vi "1_WF_Anomaly_Detection(Training).vi"() -> ()   [LabVIEW 2020]
doc: "Demonstrates the usage of Deep Learning Toolkit for solving hand written digit recognition problem with multilayer perceptron (MLP).\nDataset: MNIST http://yann.lecun.com/exdb/mnist/\nRequirements: Deep Learning Toolkit for LabVIEW"
uses:
  <vilib>/Ngene/Deep Learning Toolkit/Toolkit/NN_Train/Controls/NN_Train_Session_Data.ctl
  <vilib>/Ngene/Deep Learning Toolkit/Toolkit/NN_Train/Controls/NN_LR_Policy_Cfg.ctl
  <vilib>/Ngene/Deep Learning Toolkit/Toolkit/NN_Train/Controls/NN_LR_Policy_Type.ctl
  <vilib>/Ngene/Deep Learning Toolkit/Toolkit/NN_Train/Controls/NN_Train_Params.ctl
  <vilib>/Ngene/Deep Learning Toolkit/Toolkit/NN_Train/Controls/NN_Train_Optimizer.ctl
  <vilib>/Ngene/Deep Learning Toolkit/Toolkit/NN_Train/Controls/NN_Train_Data_Sampling.ctl
  <vilib>/Ngene/Deep Learning Toolkit/Toolkit/NN_Network/Controls/NN_Device.ctl
  <vilib>/Ngene/Deep Learning Toolkit/Toolkit/NN_Layers/Layers/Input/Controls/NN_Layer_Config_Aug(Input1D).ctl
  <vilib>/Ngene/Deep Learning Toolkit/Toolkit/NN_Layers/Layers/Input/Controls/Aug/NN_Input1D_Aug_Config.ctl
  <vilib>/Ngene/Deep Learning Toolkit/Toolkit/NN_Layers/Layers/Input/Controls/Aug/NN_Input1D_Aug_Types.ctl
  <vilib>/Ngene/Deep Learning Toolkit/Toolkit/NN_Layers/Layers/Input/Controls/Aug/Aug_Distribution_Type.ctl
  <vilib>/Ngene/Deep Learning Toolkit/Toolkit/NN_Layers/Layers/FC/Controls/NN_Layer_Config(FC).ctl
  <vilib>/Ngene/Deep Learning Toolkit/Toolkit/NN_Layers/Layers/BatchNorm/Controls/NN_BN_Params.ctl
  <vilib>/Ngene/Deep Learning Toolkit/Toolkit/NN_Activations/Controls/NN_Activation_Type.ctl
  <vilib>/Ngene/Deep Learning Toolkit/Toolkit/NN_Layers/Controls/NN_Layer_Init_Params.ctl
  <vilib>/Ngene/Deep Learning Toolkit/Toolkit/NN_Layers/Controls/NN_Layer_Weight_Init_Type.ctl
  <vilib>/Ngene/Deep Learning Toolkit/Toolkit/NN_Layers/Layers/Input/Controls/NN_Layer_Config(Input1D).ctl
  <vilib>/Ngene/Deep Learning Toolkit/Toolkit/NN_Data/Controls/NN_Data_type.ctl
  <vilib>/Ngene/Deep Learning Toolkit/Toolkit/NN_Network/Controls/NN_Save_Before_Destroy_Options.ctl
  <vilib>/Ngene/Deep Learning Toolkit/Toolkit/NN_Layers/Layers/FC/NN_Layer_Create(FC).vi
  <vilib>/Ngene/Deep Learning Toolkit/Toolkit/NN_Layers/Layers/Input/NN_Layer_Create(Input1D).vi
  <vilib>/Ngene/Deep Learning Toolkit/Toolkit/NN_Data/subVIs/Dataset/NN_Variant_to_DVR/2D/NN_Data_Variant_to_DVR(2D_SGL).vi
  <vilib>/Ngene/Deep Learning Toolkit/Toolkit/NN_Train/SubVIs/Dataset_Checks/NN_Check_Dataset(In1D_Out1D).vi
  <vilib>/Ngene/Deep Learning Toolkit/Toolkit/NN_Network/API/NN_Set_Input/1D/NN_Set_Input(1D_SGL_idx).vi
  <vilib>/Ngene/Deep Learning Toolkit/Toolkit/NN_Data/subVIs/Get_Data_Vals/2D/NN_Data_Get_ValByRef(2D_SGL_idx).vi
  <vilib>/Ngene/Deep Learning Toolkit/Toolkit/NN_Train/Loss_Functions/NN_Set_Loss(MSE).vi
  <vilib>/Ngene/Deep Learning Toolkit/Toolkit/Deep_Learning_Toolkit_by_Ngene.lvlib
  <vilib>/ptbypt/NI_PtbyPt.lvlib
panel:
  in  "Normal/Abnormal":bool=TRUE
  in  "Validation(Abnormal) dataset path":path=path "D:/working/Anomaly Detection/Validation/Abnormal"
  in  "Validation(Normal) dataset path":path=path "D:/working/Anomaly Detection/Validation/Normal"
  in  "Train(Normal) dataset path":path=path "D:/working/Anomaly Detection/Train/Normal"
  out "Anomaly Score":sgl[](graph)=[0.060092747, 0.057043016, 0.032625258, 0.00050622225, 0.07121873, 0.09103888, 0.0006431341, 0.04204446, 0.0002219677, 0.02923894, 0.060141027, 0.06411958, 0.064849555, 0.010767877, 0.033320367, 0.07314634, 0.035111904, 0.042108685, 0.01123029, 0.028102368, 0.024529666, 0.004258156, 0.024849623, 0.03586331, 0.024636567, 0.056010053, 0.006806895, 0.047554873, 0.07157735, 0.027011871, 0.025139395, 0.022341115, 0.032895457, 0.0022708364, 0.024684738, 0.006394863, 0.014353149, 0.018841192, 0.0883885, 0.048397973, 0.035732955, 0.06335908, 0.030065864, 0.03291616, 0.05862975, 0.041152924, 0.04338476, 0.00016877055, 0.009982914, 0.046630204, 0.04450816, 0.053127766, 0.03401476, 0.0791775, 0.04717928, 0.07712877, 0.058600783, 0.04143399, 0.08513886, 0.06798601, 0.051917136, 0.044983864, 0.10643387, 0.09333289, 0.10147804, 0.08439672, 0.065609634, 0.036409795, 0.073546946, 0.10952538, 0.055474997, 0.1068089, 0.084765375, 0.057112873, 0.054448366, 0.07403237, 0.06890768, 0.070016384, 0.053028703, 0.08037907, 0.04426396, 0.043441594, 0.08644903, 0.088015676, 0.047763288, 0.099104345, 0.048645973, 0.07637364, 0.014656782, 0.07575214, 0.05684656, 0.022864163, 0.017387092, 0.015441477, 0.06586057, 0.02807647, 0.018982649, 0.021074474, 0.026940286, 0.066253364, 0.018976212, 0.010368884, 0.020807803, 0.074733555, 0.019434988, 0.017290056, 0.015355766, 0.017493486, 0.033833265, 0.0105896, 0.044781208, 0.031580508, 0.009655416, 0.04107994, 0.03886822, 0.022953898, 0.015816778, 0.040687352, 0.01231581, 0.045750678, 0.0053392947, 0.021824911, 0.024692237, 0.006048307, 0.035785183, 0.0044120774, 0.024970394, 0.032739528, 0.02630835, 0.019736473, 0.10281274, 0.003404349, 0.10191603, 0.038091034, 0.03535904, 0.0002465546, 0.042997003, 0.04390773, 0.06490451, 0.09284058, 0.083866745, 0.084221035, 0.104360044, 0.04381025, 0.04932916, 0.06883395, 0.063578606, 0.05527377, 0.02474022, 0.0023239255, 0.09212524, 0.089194, 0.032360792, 0.06271982, 0.047680855, 0.050662935, 0.027425885, 0.06428027, 0.01801461, 0.04022503, 0.012174964, 0.068769336, 0.039433062, 0.03701794, 0.05450797, 0.069071054, 0.03687513, 0.0761683, 0.04485655, 0.046353817, 0.005211234, 0.03217846, 0.05994767, 0.021627009, 0.02824694, 0.025053084, 0.011249602, 0.013183653, 0.0628652, 0.033547223, 0.010532796, 0.071924865, 0.048714876, 0.025912106, 0.067157984, 0.057994485, 0.012352109, 0.03120172, 0.031498015, 0.0038321614, 0.005246043, 0.024365425, 0.07627022, 0.056759536, 0.0038585067, 0.0013263822, 0.035828173, 0.010404587, 0.06529927, 0.025035083, 0.012059271, 0.019346893, 0.026661277, 0.040283203, 0.043239236, 0.041656077, 0.011768699, 0.023633242, 0.035004884, 0.0050939023, 0.0053791404, 0.04120791, 0.0638271, 0.026579648, 0.00066304207, 0.0075542033, 0.013537571, 0.0042291284, 0.040332705, 0.020002171, 0.036556043, 0.009527139, 0.013155438, 0.01560469, 0.023518208, 0.0110270865, 0.010643028, 0.026360236, 0.02436541, 0.030391306, 0.050228402, 0.04228738, 0.0033869147, 0.036175907, 0.00611943, 0.08756912, 0.049255222, 0.020914257, 0.0037515163, 0.05814132, 0.022490084, 0.021241128, 0.036547303, 0.012504697, 0.056980252, 0.0651865, 0.04526204, 0.04104632, 0.020310044, 0.034356654, 0.0019336343, 0.064979196, 0.024666071, 0.07885355, 0.060456753, 0.057785153, 0.06992471, 0.024199843, 0.048030198, 0.061351597, 0.019730091, 0.03939289, 0.097007036, 0.0006953478, 0.008476853, 0.052414775, 0.0017266273, 0.036400378, 0.03022182, 0.06443, 0.0019540787, 0.0030147433, 0.0060815215, 0.03073597, 0.054870903, 0.0070074797, 0.029543698, 0.0017739534, 0.024344265, 0.058060706, 0.0073035955, 0.014600635, 0.0053038597, 0.024832547, 0.053949594, 0.031209469, 0.030771732, 0.036867917, 0.034106612, 0.018789113, 0.012063682, 0.024652004, 0.025159836, 0.018065631, 0.0015200973, 0.010810316, 0.02901429, 0.021046221, 0.04046935, 0.047151983, 0.073693275, 0.0008752346, 0.011598229, 0.02580303, 0.02341029, 0.014973015, 0.018914193, 0.00989604, 0.05237758, 0.043263435, 0.02045992, 0.014319763, 0.029384151, 0.03725402, 0.008532152, 0.021618426, 0.08714062, 0.012386654, 0.034504678, 0.05780665, 0.025059067, 0.037491217, 0.0035665482, 0.07386769, 0.006312445, 0.066935435, 0.08569892, 0.07021108, 0.04160881, 0.0135602355, 0.04307291, 0.017525911, 0.0078089833, 0.040077955, 0.06780583, 0.011282504, 0.027252495, 0.0052479506, 0.08056086, 0.051447213, 0.07204753, 0.045395255, 0.009712577, 0.00199759, 0.0043674707, 0.02886641, 0.057467997, 0.0033851862, 0.018882632, 0.035472095, 0.07547408, 0.05349207, 0.013515651, 0.023959875, 0.059220076, 0.028184414, 0.0042169094, 0.0054979324, 0.021413028, 0.00018376112, 0.04798007, 0.0035876632, 0.00085502863, 0.015411198, 0.03357798, 0.0141349435, 0.025293052, 0.06722516, 0.035633385, 0.03246671, 0.0073210597, 0.0033890605, 0.051241398, 0.031478405, 0.0120385885, 0.04314059, 0.0051404834, 0.0022211075, 0.060732722, 0.03339243, 0.027571142, 0.03379011, 0.02301824, 0.023383796, 0.023100555, 0.0034759045, 0.004920721, 0.014518559, 0.005325496, 0.06771225, 0.029369414, 0.037244976, 0.028220832, 0.035060287, 0.019271076, 0.045505702, 0.06212762, 0.037652284, 0.012569755, 0.012304664, 0.046938777, 0.029604435, 0.016992986, 0.02305895, 0.0012228787, 0.014539182, 0.016175747, 0.041780204, 0.032874674, 0.04862517, 0.07770675, 0.04169628, 0.058294393, 0.053397845, 0.07256114, 0.033954605, 0.060890388, 0.0009793043, 0.109390326, 0.048723236, 0.006696999, 0.013124093, 0.03138551, 0.02865538, 0.0050074756, 0.026816845, 0.0021244586, 0.01151374, 0.010649353, 0.036117435, 0.01668498, 0.041314363, 0.03689885, 0.011788726, 0.04051286, 0.048635185, 0.0010183454, 0.03554952, 0.049126625, 0.049170673, 0.04226947, 0.02651894, 0.026122332, 0.00902319, 0.014714181, 0.053105295, 0.03526801, 0.045228064, 0.005509317, 0.012253821, 0.008698344, 0.02798599, 0.03927982, 0.009805262, 0.023320377, 0.026049614, 0.030642271, 0.0005450845, 0.0044911504, 0.013210893, 0.025141537, 0.027490556, 0.011119723, 0.027630031, 0.013084769, 0.037715316, 0.01857531, 0.0246706, 0.028110027, 0.017253816, 0.055761278, 0.02272594, 0.02098006, 0.023195267, 0.008237243, 0.034432173, 0.03778249, 0.0037900805, 0.016308367, 0.01734817, 0.05744642, 0.044672668, 0.014907718, 0.02106911, 0.022406042, 0.0028811693, 0.048549235, 0.07803196, 0.043880284, 0.007881284, 0.014288545, 0.040141463, 0.037219048, 0.025383472, 0.028543562, 0.037507176, 0.06284988, 0.06856242, 0.045178384, 0.06358957, 0.06256491, 0.09023467, 0.066772714, 0.03930801, 0.089330375, 0.045202382, 0.0012217015, 0.03294455, 0.074084684, 0.031060789, 0.07108601, 0.06460565, 0.03949655, 0.02086892, 0.022628829, 0.0531967, 0.043416634, 3.7267804e-05, 0.0069933236, 0.007908642, 0.00840199, 0.010333836, 0.08059165, 0.018291354, 0.00983268, 0.02023545, 0.052577674, 0.028196096, 0.04909426, 0.06960064, 0.018643081, 0.018747628, 0.052239835, 0.03520423, 0.020172, 0.035363674, 0.03190261, 0.03205198, 0.027214646, 0.0010645986, 0.033943415, 0.06383264, 0.026733339, 0.023622096, 0.006123543, 0.034471333, 0.0123743415, 0.037702322, 0.022325516, 0.0033456087, 0.015103638, 0.038256645, 0.00042706728, 0.032328308, 0.0027711987, 0.029803038, 0.029901206, 0.016103625, 0.040743887, 0.020637393, 0.032048166, 0.017939508, 0.03243172, 0.0057141185, 0.012813866, 0.013404548, 0.012252271, 0.0017794967, 0.0056546926, 0.04450822, 0.05620414, 0.013124406, 0.018638313, 0.022311866, 0.030828714, 0.06490421, 0.046281636, 0.057371557, 0.03398019, 0.01053822, 0.022645772, 0.050679624, 0.02049148, 0.02902317, 0.059186637, 0.031636357, 0.0341025, 0.003514707, 0.034976006, 0.050084323, 0.06393728, 0.027762264, 0.030045897, 0.0034492016, 0.04939601, 0.026292771, 0.03334993, 0.016023219, 0.055217057, 0.08875525, 0.034162715, 0.03684184, 0.09832852, 0.0032533929, 0.04504199, 0.072000064, 0.008023124, 0.03721671, 0.07505199, 0.07275631, 0.061018378, 0.033247128, 0.04330583, 0.016284913, 0.07300937, 0.05863276, 0.060104758, 0.015596688, 0.020811826, 0.056227475, 0.109434426, 0.050217718, 0.011233985, 0.016816437, 0.014317572, 0.017227054, 0.01705122, 0.067214906, 0.007261336, 0.0041286945, 0.004626453, 0.008798957, 0.033632636, 0.011648834, 0.0064768195, 0.015599787, 0.010294795, 0.03991133, 0.022496164, 0.01535368, 0.010416925, 0.014266193, 0.004371822, 0.05693829, 0.03694272, 0.01812011, 0.008884549, 0.014544427, 0.01466769, 0.014502704, 0.03141892, 0.004409075, 0.01927048, 0.0057350993, 0.010116279, 0.010567248, 0.02657038, 0.03631872, 0.02690959, 0.004686594, 0.033815324, 0.016802311, 0.0529083, 0.018151581, 0.04130584, 0.008548856, 0.049080312, 0.0076634884, 0.021098077, 0.011823714, 0.0067802668, 0.018489897, 0.022878766, 0.041176736, 0.042533934, 0.06584221, 0.02490908, 0.054923594, 0.052935958, 0.01268357, 0.06410545, 0.05014521, 0.046426475, 0.020729423, 0.026006311, 0.04061067, 0.032135606, 0.01457727, 0.04491949, 0.08099672, 0.020792186, 0.018885136, 0.013119906, 0.00464952, 0.036944523, 0.022346139, 0.0232165, 0.048607357, 0.06732133, 0.026639529, 0.042294167, 0.059899196, 0.04408887, 0.056200996, 0.022303723, 0.026353091, 0.025170714, 0.011349812, 0.027633563, 0.07789123, 0.039173394, 0.026246369, 0.0060180426, 0.058868974, 0.060914278, 0.041833967, 0.06189263, 0.031127632, 0.020099223, 0.02997011, 0.041916907, 0.009172618, 0.010260463, 0.026746035, 0.0043724775, 0.017262697, 0.026671827, 0.00696671, 0.07369858, 0.0056867003, 0.021373391, 0.014488459, 0.018270016, 0.0076046586, 0.025081098, 0.05353415, 0.0067960024, 0.0021197796, 0.0688144, 0.013996065, 0.002437532, 0.016689777, 0.031236827, 0.0032956004, 0.0065782666, 0.029214263, 0.034022868, 0.028901994, 0.017384768, 0.067723095, 0.049763322, 0.022492647, 0.03597647, 0.0014654398, 0.041612327, 0.019034028, 0.036304176, 0.02889496, 0.061680317, 0.02313286, 0.05067444, 0.040518403, 0.02105838, 0.05028844, 0.0042199492, 0.031202018, 0.008577466, 0.01362288, 0.051632464, 0.037617743, 0.015216768, 0.09837359, 0.017223299, 0.04835391, 0.05309844, 0.026347697, 0.028072476, 0.03628832, 0.0038926005, 0.011207044, 0.0026324391, 0.049726874, 0.0274854, 0.032975346, 0.03847137, 0.05839902, 0.015199244, 0.03004378, 0.04979439, 0.04324563, 0.046655342, 0.021768764, 0.03619662, 0.010923855, 0.014889538, 0.061536007, 0.009047002, 0.040081657, 0.032270912, 0.011951536, 0.0033479854, 0.029726982, 0.014376685, 0.07876404, 0.033536434, 0.048506677, 0.014585793, 0.028419942, 0.058252603, 0.019356698, 0.031891465, 0.027893305, 0.01727137, 0.024498105, 0.03793639, 0.021569252, 0.021141887, 0.031154454, 0.048297763, 0.045414805, 0.024651527, 0.061146736, 0.0019143224, 0.02575016, 0.04922664, 0.0015360117, 0.03846699, 0.0061448216, 0.03153044, 0.023596048, 0.0183779, 0.059889495, 0.02276653, 0.0115686655, 0.0039538145, 0.0136953, 0.046172798, 0.00835675, 0.019180536, 0.009189963, 0.016337872, 0.012678146, 0.014078021, 0.008511364, 0.011597872, 0.010782659, 0.0040802956, 0.016313553, 0.019533575, 0.027357697, 0.033422947, 0.020239234, 0.049649775, 0.007699847, 0.06390226, 0.002970636, 0.026395619, 0.017627835, 0.019885242, 0.033176243, 0.01590389, 0.019070506, 0.018345714, 0.0038775206, 0.035709083, 0.0021954775, 0.018336892, 0.051371634, 0.030016303, 0.029429913, 0.030059338, 0.064861536, 0.038681805, 0.014020205, 0.031060219, 0.009667695, 0.027311891, 0.012509435, 0.027186513, 0.03732568, 0.033010572, 0.013314575, 0.0018598139, 0.027742833, 0.04039496, 0.0032858849, 0.029230148, 0.058380455, 0.02820637, 0.0710767, 0.028457515, 0.06434338, 0.006146811, 0.031927288, 0.019665599, 0.016479976, 0.019756787, 0.029963478, 0.024598971, 0.036068127, 0.034127593, 0.007751018, 0.026875377, 0.0043821633, 0.028044999, 0.023972422, 0.0101952255, 0.0024086833, 0.050703526, 0.0061364174, 0.017236412, 0.04354602, 0.06092578, 0.030829191, 0.020911515, 0.0019962192, 0.039640963, 0.011587381, 0.011074901, 0.011200011, 0.009899557, 0.007934749, 0.0070021152, 0.03636366, 0.025456786, 0.0021848083, 0.035301924, 0.025167406, 0.002292931, 0.018001676, 0.029745579, 0.025209725, 0.018230438, 0.04587239, 0.036272824, 0.013392806, 0.014877796, 0.022945702, 0.050283194, 0.0076546073, 0.05172223, 0.064860165, 0.02660191, 0.03967929, 0.028658807, 0.01357156, 0.0019970536, 0.04909706, 0.011058211, 0.0065134764, 0.037633598, 0.05778092, 0.031118214, 0.011135042, 0.026689708, 0.0594669, 0.0330171, 0.46308094, 0.40537137, 0.41881543, 0.39853013, 0.39663595, 0.41779327, 0.3711896, 0.35427624, 0.3763141, 0.3562011, 0.36535013, 0.27024323, 0.3030228, 0.32000816, 0.27570146, 0.23469242, 0.19539478, 0.26820946, 0.18958178, 0.20020002, 0.19895002, 0.2031722, 0.15438448, 0.19178395, 0.09444921, 0.074550316, 0.109781526, 0.117275275, 0.08901222, 0.06565887, 0.008233057, 0.024207637, 0.023363285, 0.02861242, 0.063968666, 0.085702434, 0.0734206, 0.085044876, 0.09044993, 0.15952384, 0.106506884, 0.111953944, 0.18576512, 0.24552834, 0.17271072, 0.22364199, 0.2632353, 0.26729608, 0.27913588, 0.2879197, 0.3019418, 0.31883794, 0.34263408, 0.3339213, 0.37668836, 0.35255224, 0.36873883, 0.3697074, 0.36853063, 0.43723994, 0.4041955, 0.40559894, 0.4054047, 0.42701077, 0.4128943, 0.465872, 0.48269498, 0.45807642, 0.45683855, 0.4586808, 0.47161806, 0.4765666, 0.4903825, 0.54455686, 0.48940068, 0.4847442, 0.47246432, 0.5273197, 0.50743175, 0.49895048, 0.54400766, 0.5125568, 0.5317018, 0.53908825, 0.51740736, 0.49215025, 0.46106368, 0.5066986, 0.45588142, 0.47801656, 0.49033332, 0.47162968, 0.48650628, 0.46554434, 0.42119676, 0.44083905, 0.3966776, 0.424111, 0.38918126, 0.3865584, 0.3825484, 0.35784245, 0.38309276, 0.36913866, 0.31185722, 0.30031657, 0.29074007, 0.29277796, 0.27721256, 0.30074963, 0.2617998, 0.25614235, 0.24356678, 0.24000305, 0.1939761, 0.21740982, 0.17069659, 0.12884587, 0.1654735, 0.10129453, 0.11253221, 0.08823912, 0.09139761, 0.061363183, 0.007372923, 0.018441636, 0.029024683, 0.030053724, 0.03293188, 0.07232845, 0.06228201, 0.0626775, 0.06774281, 0.14145167, 0.10842833, 0.13371754, 0.1754123, 0.20848632, 0.2327654, 0.17804009, 0.255733, 0.24676377, 0.19095165, 0.25900787, 0.27888352, 0.27582014, 0.33042967, 0.3364432, 0.3330053, 0.37317473, 0.3458109, 0.36236846, 0.38359535, 0.40375018, 0.413059, 0.4453684, 0.41684794, 0.45065308, 0.4877693, 0.46055377, 0.4286015, 0.49897814, 0.49796456, 0.46430838, 0.46328366, 0.4589039, 0.48185307, 0.5112523, 0.5091743, 0.50040674, 0.4602269, 0.5490465, 0.48672992, 0.49818873, 0.5526335, 0.5185267, 0.52889794, 0.49323076, 0.4622165, 0.5050069, 0.52549446, 0.53211826, 0.5107923, 0.47318977, 0.47224635, 0.48238593, 0.48093635, 0.43763262, 0.4665349, 0.49588674, 0.3934558, 0.40964812, 0.46183956, 0.40744114, 0.3582679, 0.36755997, 0.35740298, 0.3827818, 0.38228112, 0.323766, 0.35789853, 0.36108774, 0.25618678, 0.33311367, 0.23510003, 0.26440957, 0.230688, 0.24481863, 0.217704, 0.17933613, 0.20121786, 0.17480981, 0.15428665, 0.14260572, 0.10653743, 0.17568992, 0.09242158, 0.09771779, 0.106368616, 0.056124955, 0.04469486, 0.008346185, 0.013324438, 0.06648501, 0.03256286, 0.076318845, 0.098160565, 0.12020953, 0.12958886, 0.15207501, 0.109490156, 0.184427, 0.18866935, 0.23817441, 0.21397722, 0.2280165, 0.22041285, 0.2009595, 0.23724687, 0.2935543, 0.302481, 0.30630094, 0.3419844, 0.36041856, 0.373222, 0.36745453, 0.3785169, 0.41459596, 0.3870151, 0.37493777, 0.4352523, 0.40611255, 0.41030478, 0.43105018, 0.45878255, 0.40033156, 0.47421598, 0.4906655, 0.5241343, 0.48030663, 0.49060512, 0.5424207, 0.49666417, 0.46434093, 0.46581465, 0.49979085, 0.45077455, 0.47974205, 0.49341488, 0.55592084, 0.50985223, 0.46209037, 0.5000891, 0.5022733, 0.48341233, 0.4983245, 0.45872438, 0.4922198, 0.47661215, 0.4807518, 0.48118544, 0.45343256, 0.4768914, 0.44529247, 0.48953515, 0.45412433, 0.43775922, 0.40525293, 0.4392395, 0.42524123, 0.39710408, 0.4001888, 0.3877796, 0.3678217, 0.39252263, 0.31871283, 0.36604935, 0.32473528, 0.26952988, 0.25438154, 0.2668668, 0.2545808, 0.2627398, 0.23875633, 0.24298686, 0.19150075, 0.14178625, 0.20359081, 0.1495145, 0.11560753, 0.054015756, 0.05677551, 0.058844447, 0.03357549, 0.026502363, 0.0048035905, 0.009981088, 0.013024547, 0.0006883219, 0.040967263, 0.06830982, 0.08867513, 0.08777779, 0.09626874, 0.13023503, 0.12196019, 0.16031587, 0.16264138, 0.17573929, 0.20352799, 0.23217982, 0.25994548, 0.24100539, 0.2453689, 0.27634645, 0.2999044, 0.32158947, 0.33817136, 0.34101284, 0.31473905, 0.3742748, 0.37150532, 0.40105838, 0.41667008, 0.43249565, 0.39946848, 0.43296075, 0.42731118, 0.44064432, 0.4375021, 0.46769643, 0.4667257, 0.4741361, 0.4748779, 0.50883967, 0.5422015, 0.49947774, 0.44423503, 0.50826883, 0.5058737, 0.5043425, 0.47624505, 0.53109246, 0.5006827, 0.54043067, 0.5234734, 0.5252645, 0.4885658, 0.5095222, 0.48674482, 0.52490056, 0.47955245, 0.43071008, 0.48607934, 0.47437918, 0.4550978, 0.45574284, 0.42089272, 0.49345458, 0.42376143, 0.4433015, 0.45101416, 0.4033786, 0.41903245, 0.36262196, 0.41138083, 0.41466612, 0.36319888, 0.40269518, 0.35782278, 0.3430887, 0.3391332, 0.32773423, 0.30320036, 0.27438104, 0.25276166, 0.18347871, 0.29438615, 0.22050172, 0.23142046, 0.20882559, 0.17307681, 0.21495005, 0.17710039, 0.13610429, 0.120277286, 0.123796955, 0.1116191, 0.07928431, 0.03175263, 0.011327803, 0.02305593, 0.015505847, 0.017093897, 0.06495239, 0.05048629, 0.0974765, 0.055347815, 0.072373316, 0.1392326, 0.14378516, 0.18232095, 0.17093965, 0.15067703, 0.21434084, 0.21461153, 0.27226913, 0.2511737, 0.251593, 0.256446, 0.24557245, 0.30787134, 0.32068497, 0.3608482, 0.3207535, 0.41698748, 0.36563152, 0.33165878, 0.40249974, 0.41461235, 0.4340843, 0.37705785, 0.38703918, 0.4186424, 0.4576856, 0.48705655, 0.4518482, 0.43026507, 0.48211175, 0.47307044, 0.48190945, 0.5136361, 0.4808041, 0.49484515, 0.49358463, 0.5716697, 0.49971783, 0.47741067, 0.088213146, 0.004971981, 0.0018055439, 0.03895092, 0.00883013, 0.008856475, 0.03728193, 0.012614429, 0.0017704964, 0.015758514, 0.007663667, 0.011581898, 0.0005093813, 0.024503171, 0.027090132, 0.002755165, 0.03364426, 0.036851823, 0.04900217, 0.045261025, 0.05881405, 0.042640567, 0.018819094, 0.03572011, 0.040177405, 0.021710753, 0.009258747, 0.026422977, 0.035487354, 0.0016648173, 0.038206995, 0.04202175, 0.01727885, 0.06741437, 0.017207712, 0.023454756, 0.0004569292, 0.053476125, 0.025311321, 0.010994464, 0.0130132735, 0.024535358, 0.031835288, 0.022631496, 0.008303836, 0.031224988, 0.022085734, 0.007815503, 0.005466588, 0.027604412, 0.021293122, 0.010265693, 0.0056704953, 0.014358774, 0.020382062, 0.0059206784, 0.030814424, 0.022508532, 0.04299441, 0.0435777, 0.0064103305, 0.011587173, 0.020177037, 0.006169319, 0.040371984, 0.019659698, 0.0133242905, 0.016918123, 0.011550605, 0.044745088, 0.014496326, 0.024675846, 0.030195236, 0.0009198189, 0.013777554, 0.038612247, 0.023512006, 0.054900587, 0.013043821, 0.01527369, 0.031131208, 0.016245365, 0.017644405, 0.013945162, 0.044774413, 0.04253936, 0.019254744, 0.0065425634, 0.005466819, 0.009824753, 0.011426508, 0.018061817, 0.04737252, 0.06586492, 0.04055369, 0.020852983, 0.05214429, 0.025059223, 0.035581887, 0.01780492, 0.052277386, 0.049828768, 0.015147746, 0.037875116, 0.0230788, 0.0071218014, 0.037825286, 0.0048089623, 0.02847135, 0.026385725, 0.02560842, 0.01971668, 0.023034811, 0.04307258, 0.048989415, 0.020333767, 0.040479302, 0.0028678179, 0.021646798, 0.03186208, 0.07786274, 0.02560246, 0.034244478, 0.008883357, 0.049423993, 0.009867549, 0.04767102, 0.024399936, 0.019941986, 0.01684466, 0.027478337, 0.0059705973, 0.0019535124, 0.05311224, 0.034656763, 0.00039172173, 0.004858911, 0.034396872, 0.030774772, 0.011311963, 0.022923708, 0.0012369007, 0.0124548, 0.011488877, 0.009216271, 0.031239416, 0.015381483, 0.03874389, 0.059431456, 0.029807314, 0.009363398, 0.0037425607, 0.060222745, 0.017440826, 0.047270715, 0.0257079, 0.021419376, 0.036061525, 0.0357503, 0.0034706295, 0.0016235709, 0.0055321753, 0.0393759, 0.043245614, 0.06003958, 0.0044566393, 0.050515473, 0.00054210424, 0.016351223, 0.007889926, 0.031197608, 0.04330963, 0.004803598, 0.015920639, 0.0041899085, 0.008691192, 0.03660202, 0.01127708, 0.008189201, 0.03909087, 0.0120411515, 0.025409162, 0.038364112, 0.008698046, 0.01937294, 0.029666424, 0.0012822747, 0.011394918, 0.05077547, 0.016393542, 0.010116637, 0.014395237, 0.012369573, 0.021274984, 0.004901111, 0.007912874, 0.003569305, 0.03259158, 0.003264606, 0.0066278577, 0.008854747, 0.013671577, 0.013440728, 0.031002462, 0.013184428, 0.0018249154, 0.01794827, 0.022874594, 0.010919929, 0.006907344, 0.02766782, 0.0077005625, 0.002740562, 0.011553168, 0.009389579, 0.036827743, 0.04146391, 0.0017961264, 0.016017973, 0.054489374, 0.034730136, 0.0070807934, 0.0073878765, 0.0067406893, 0.040196896, 0.03732884, 0.0125771165, 0.0036627352, 0.0033930838, 0.037597805, 0.040892392, 0.00045531988, 0.026380181, 0.02078113, 0.020073548, 0.031786785, 0.0096321255, 0.02771762, 0.06532389, 0.0065064467, 0.017363671, 0.02354199, 0.00056259707, 0.0478601, 0.0072613284, 0.031705298, 0.033976957, 0.030823603, 0.014133573, 0.05249217, 0.008479834, 0.013263732, 0.023093611, 0.05352822, 0.027314872, 0.021412313, 0.051763356, 0.029191256, 0.04939753, 0.014547646, 0.021043122, 0.002128005, 0.033852935, 0.002283156, 0.018767834, 0.0082476735, 0.057578743, 0.008703709, 0.02977264, 0.045514107, 0.0064259768, 0.024143219, 0.00058704615, 0.033961773, 0.017675817, 0.020857394, 0.0069206357, 0.03106147, 0.028582215, 0.0061181784, 0.03827566, 0.00752455, 0.013832986, 0.0048981905, 0.002655983, 0.0075912476, 0.01634401, 0.005961001, 0.0039411783, 0.03264141, 0.019039273, 0.0056370497, 0.028300107, 0.048362434, 0.011524618, 0.019236028, 0.045313597, 0.016815364, 0.0032744408, 0.02021724, 0.008698344, 0.039801657, 0.011592567, 0.0049014688, 0.0033550262, 0.010494053, 0.041498303, 0.0019505024, 0.0075753927, 0.062099755, 0.023397207, 0.015686214, 0.00673151, 0.051026106, 0.0130741, 0.024833083, 0.0071051717, 0.013831437, 0.0013015866, 0.013917923, 0.05097398, 0.011403829, 0.033909917, 0.028137237, 0.020659775, 0.00306499, 0.00961405, 0.023068905, 0.049004987, 0.027510718, 0.002244234, 0.0083640665, 0.009853184, 0.05006399, 0.03839422, 0.013824053, 0.015105287, 0.04802212, 0.03085161, 0.019875668, 0.051975526, 0.057991803, 0.04961741, 0.006469205, 0.02126655, 0.0066388845, 0.02709493, 0.023671597, 0.029837668, 0.015945435, 0.021256477, 0.029453754, 0.0351713, 0.042717934, 0.009555817, 0.016029775, 0.03376788, 0.026853442, 0.011680543, 0.0005262494, 0.038778007, 0.06310338, 0.016598046, 0.03478545, 0.0012992024, 0.008657217, 0.0058189034, 0.048874795, 0.009764671, 0.021235585, 0.020060122, 0.022887468, 0.0080522895, 0.009318709, 0.039521396, 0.028623164, 0.09320015, 0.017876625, 0.022607267, 0.0048077703, 0.046610177, 0.02415967, 0.04211378, 0.0011832714, 0.023078442, 0.050397158, 0.03108728, 0.019585967, 0.0035603046, 0.047453284, 0.024101138, 0.0014281869, 0.045340538, 0.044525564, 0.0016590953, 0.0141605735, 0.026108742, 0.03748089, 0.02467233, 0.0008909106, 0.007987499, 0.0076344013, 0.013087571, 0.009227753, 0.00024867058, 0.0014616251, 0.014864981, 0.005414307, 0.036056936, 0.043343246, 0.022282362, 0.038059294, 0.02708751, 0.04222727, 0.03550881, 0.0072185993, 0.045993686, 0.0014115572, 0.005900383, 0.048186183, 0.001932621, 0.025222749, 0.036120057, 0.00844875, 0.03433752, 0.017096907, 0.018903464, 0.0065089613, 0.038067468, 0.0030327663, 0.036202714, 0.00499543, 0.02893943, 0.01747746, 0.040883083, 0.012874626, 0.028355196, 0.04346603, 0.028442562, 0.00061137974, 0.03607595, 0.024472505, 0.065160066, 0.060543686, 0.04700324, 0.009227753, 0.05112952, 0.004482627, 0.0035113692, 0.029662192, 0.012503326, 0.013845503, 0.030131519, 0.0039847493, 0.036280334, 0.0009837747, 0.05604273, 0.054259896, 0.06530589, 0.016978383, 0.011705279, 0.049054146, 0.088528395, 0.03491634, 0.05571854, 0.06517869, 0.004814744, 0.023220122, 0.060379803, 0.00031524897, 0.10123885, 0.0016469955, 0.014386773, 0.08758116, 0.024338484, 0.061982095, 0.036061227, 0.011523306, 0.032522142, 0.003698945, 0.005343735, 0.0070099235, 0.05074066, 0.0031623244, 0.00067567825, 0.052962124, 0.0416373, 0.020732641, 0.0266639, 0.0035790205, 0.031341136, 0.015119493, 0.004871011, 0.06593907, 0.0006110072, 0.0050964355, 0.041249037, 0.07265675, 0.035296798, 0.04400152, 0.027931035, 0.0001667738, 0.026423872, 0.0020712614, 0.007370651, 0.009222269, 0.01358521, 0.0327062, 0.010226071, 0.026578546, 0.002227068, 0.017990053, 0.03734836, 0.027296841, 0.009459108, 0.04408452, 0.003448695, 0.0073421896, 0.038420737, 0.0027022362, 0.05409248, 0.0046785176, 0.08546027, 0.05786114, 0.008815475, 0.028135657, 0.031370837, 0.051256217, 0.031129003, 0.029532269, 0.016701564, 0.010883853, 0.061577633, 0.05408442, 0.023234189, 0.0480057, 0.031064928, 0.022515267, 0.03847283, 0.03286642, 0.08277196, 0.0374375, 0.0899438, 0.03274271, 0.022776306, 0.026878774, 0.03246647, 0.04005915, 0.08015013, 0.022920787, 0.0754078, 0.051899612, 0.07204807, 0.058280647, 0.019641161, 0.018536925, 0.0564667, 0.058317184, 0.037928164, 0.016976058, 0.07734418, 0.04926735, 0.062363625, 0.029133976, 0.015916407, 0.032779396, 0.041973352, 0.106060684, 0.055249095, 0.06885409, 0.08311707, 0.076545656, 0.039178014, 0.079859436, 0.08364719, 0.0040640235, 0.041940868, 0.049610257, 0.04788947, 0.068831384, 0.07340938, 0.01848793, 0.031992972, 0.06386858, 0.031677544]
  out "Loss Chart":dbl(graph)=5.313800277709961
  out "Input & Reconstructed Signals":sgl[][](graph)=[[-222.74225, -218.17032, -207.99007, -195.96149, -208.3725, -208.32933, -181.28564, -186.49068, -170.93327, -172.37735, -174.03384, -168.9887, -163.1639, -143.94429, -142.87688, -145.95512, -130.10686, -125.066086, -110.69527, -94.05543, -99.487114, -85.378044, -84.92391, -62.912807, -58.16722, -42.95759, -50.353653, -29.626831, -16.181437, -18.957151, -11.726545, -4.4781327, 5.73491, 6.305001, 19.604338, 19.825233, 32.724754, 41.481888, 66.09324, 64.175514, 68.57591, 82.886185, 82.33581, 90.459885, 104.07114, 107.076706, 114.57234, 111.31949, 120.47591, 135.99124, 142.20195, 150.75066, 152.40355, 169.48259, 167.80302, 180.9909, 182.06418, 183.46416, 199.23332, 200.15663, 201.34012, 204.23613, 223.54413, 224.7199, 230.75473, 230.49521, 229.5863, 225.93834, 237.97127, 249.4861, 239.15399, 253.87413, 250.74368, 246.02708, 247.06761, 253.20776, 253.17784, 254.40393, 250.80688, 257.85098, 249.42336, 248.986, 258.82776, 258.72375, 248.1032, 259.22504, 245.67503, 250.64967, 233.91762, 246.4205, 239.48317, 228.68741, 224.4929, 213.49403, 229.64653, 216.97835, 210.95584, 207.37787, 204.46567, 209.58081, 193.4343, 186.56854, 173.80612, 191.45605, 172.90439, 166.62961, 153.03462, 146.52158, 152.59998, 135.69849, 142.50749, 132.61932, 116.0027, 121.219185, 113.72837, 102.70894, 86.20397, 73.035034, 72.404205, 56.939835, 61.521427, 57.797977, 38.953865, 38.651592, 20.931557, 20.541101, 7.927105, -1.857486, -8.234004, -14.576754, -42.195057, -26.257044, -57.579845, -50.18185, -57.20617, -56.340828, -74.15928, -82.05786, -94.53708, -108.44174, -113.72801, -121.01305, -132.80641, -125.23446, -133.27899, -144.68015, -150.13885, -154.38571, -153.29765, -154.15775, -181.47005, -186.52657, -178.64659, -191.21277, -192.8834, -198.6391, -197.86221, -211.26726, -204.4835, -213.89401, -211.24199, -228.42465, -224.98393, -227.76431, -234.84192, -241.21706, -235.89003, -247.72038, -242.12556, -244.40492, -235.97069, -243.88284, -251.50743, -243.03049, -245.09926, -244.57274, -241.2599, -241.48407, -252.92764, -245.17133, -238.68788, -251.98196, -244.97157, -237.8189, -245.5579, -240.95868, -227.6045, -229.24841, -226.43953, -216.43971, -210.90096, -202.47229, -222.78485, -186.5377, -196.76604, -191.59833, -195.07877, -183.9371, -192.07182, -176.88843, -168.25423, -154.95676, -147.2013, -157.26797, -151.73741, -144.87746, -125.575516, -127.35198, -106.318825, -109.222534, -99.509, -83.7101, -71.0815, -85.33911, -71.36087, -65.893005, -53.15098, -49.73499, -31.360151, -28.559479, -16.66655, -15.473487, -12.997305, 1.8251256, 11.40437, 16.3265, 24.154327, 35.606457, 43.0477, 52.173916, 64.614815, 50.091026, 68.49286, 83.802216, 84.02866, 111.01659, 109.021255, 109.41942, 110.45963, 132.03392, 130.43762, 136.61786, 146.77135, 141.47887, 164.15526, 172.12476, 173.34288, 177.85112, 178.39441, 187.0456, 184.30406, 204.475, 199.35986, 216.92485, 216.82962, 220.26843, 227.02193, 219.64795, 228.72723, 235.04437, 227.93523, 235.2943, 251.52168, 230.56688, 230.28555, 246.57956, 235.85439, 245.3761, 244.85324, 253.5432, 238.09102, 239.52354, 240.01956, 245.45663, 224.43098, 238.3218, 242.53049, 234.42575, 238.16263, 244.33456, 229.99286, 222.33585, 224.47293, 214.36018, 204.25209, 221.33026, 202.85478, 197.5517, 194.13441, 193.49062, 190.78471, 194.79648, 178.04164, 174.46425, 173.88483, 170.59447, 155.51657, 151.6689, 160.43265, 133.16353, 120.313614, 131.73006, 127.82358, 112.12727, 116.97847, 100.80648, 101.73941, 92.375046, 70.22938, 64.976776, 62.76962, 56.803253, 45.507805, 35.939037, 39.247715, 24.33158, 0.6862514, 16.652798, -2.2811224, -15.793596, -15.8541765, -26.51789, -24.584028, -50.848244, -42.55499, -64.7845, -76.96774, -80.69066, -81.50612, -82.214455, -76.06251, -97.80621, -102.67416, -117.37871, -130.9934, -124.38781, -134.70059, -136.1395, -160.4546, -159.94733, -170.8914, -170.49487, -163.02899, -170.40057, -175.11182, -188.36794, -200.27232, -192.09244, -200.37183, -208.6733, -222.59378, -221.1581, -208.91624, -221.27037, -233.09282, -228.52426, -223.62794, -225.72049, -224.30087, -231.31589, -244.79521, -233.85896, -236.36522, -240.81868, -245.89871, -234.92761, -244.63034, -254.69405, -246.87201, -245.632, -235.36295, -235.34663, -222.42206, -240.83482, -228.47073, -239.79373, -225.80627, -225.17307, -236.33586, -210.86581, -222.13707, -204.05037, -202.79561, -210.09212, -194.61586, -196.67421, -192.46097, -189.96446, -182.71811, -159.90907, -163.83134, -156.4212, -152.82701, -145.18553, -142.97495, -152.28137, -119.96937, -119.36346, -118.66327, -111.76688, -96.49469, -93.69493, -89.52168, -80.86585, -79.25349, -68.0306, -60.19782, -46.37275, -40.83008, -29.36996, -14.710381, -15.432893, -3.7693458, 2.975483, 15.494673, 13.909105, 28.293694, 21.835033, 55.53368, 48.893578, 46.48728, 55.70978, 67.77252, 60.80271, 76.32179, 88.99605, 90.50987, 94.43671, 106.95585, 120.02818, 122.324394, 134.95546, 140.37572, 140.82928, 154.20308, 162.15244, 156.72441, 171.01189, 179.79039, 185.32095, 188.94467, 190.44455, 195.14935, 195.84557, 201.5314, 215.06528, 214.86432, 221.09473, 215.16223, 220.14091, 218.23239, 216.48337, 235.26715, 225.88673, 235.99689, 238.5719, 241.35416, 235.57082, 235.56212, 240.77061, 232.04602, 245.15775, 241.46873, 245.19121, 234.93965, 246.65167, 232.18193, 229.51906, 240.74641, 228.17908, 243.7827, 222.78577, 220.80478, 228.76686, 218.34306, 208.93628, 222.90779, 211.14961, 210.31401, 198.15643, 184.21286, 182.95856, 192.45786, 179.02342, 173.42255, 172.82852, 156.34818, 143.75232, 145.94873, 148.58849, 141.05075, 128.36604, 122.587425, 118.947975, 111.46954, 102.35828, 89.31603, 80.74502, 79.15719, 67.29851, 60.344425, 46.02368, 44.214546, 43.126076, 23.440712, 26.351429, 28.986792, 13.693309, -4.100324, -1.4545894, -18.980642, -25.345358, -27.239172, -30.44854, -38.79092, -53.80721, -59.13999, -56.408943, -65.75839, -73.418076, -80.97648, -88.88013, -112.94199, -105.18992, -110.11984, -119.57651, -134.29865, -135.16707, -146.66261, -158.06415, -152.07434, -158.09943, -172.13757, -173.80902, -175.72128, -167.67273, -189.09662, -178.78752, -197.81151, -196.0955, -192.01358, -219.79984, -214.736, -206.49069, -216.98965, -227.15312, -224.72984, -233.68855, -232.39812, -230.24294, -234.98486, -224.0984, -234.8225, -243.9188, -236.45491, -230.68727, -231.1437, -234.69513, -248.33853, -233.36702, -245.53156, -232.81451, -228.37639, -233.3486, -230.20467, -234.57709, -226.49945, -226.61292, -225.99713, -211.07803, -205.391, -212.37015, -207.6868, -202.96515, -197.08112, -184.583, -184.7324, -177.51082, -178.32475, -178.91083, -170.72502, -158.71689, -160.44205, -152.63445, -139.3952, -140.00728, -133.1754, -135.72353, -120.00577, -109.65977, -99.37505, -101.09705, -93.58898, -94.4278, -74.54496, -72.649734, -63.516018, -60.234425, -43.147907, -27.41874, -32.84095, -24.517958, -1.8411535, -16.739185, 0.970077, 15.360015, 4.0744505, 22.612011, 39.61248, 46.741516, 51.84441, 52.859314, 62.9534, 56.33162, 85.20225, 89.43186, 97.22514, 93.7432, 102.19484, 117.89459, 137.62425, 130.37225, 127.73616, 135.55594, 141.43622, 148.61449, 154.57228, 172.85158, 164.22272, 168.99089, 174.63034, 180.91174, 176.00818, 191.67572, 195.23444, 201.74394, 199.84924, 215.97873, 215.63907, 217.52487, 219.70006, 223.74388, 222.15076, 212.1748, 219.37375, 226.05116, 234.45229, 230.50934, 238.96025, 240.12065, 245.14055, 237.02182, 233.93509, 237.42358, 236.1321, 235.54385, 231.22311, 227.92351, 228.9817, 235.12479, 224.20432, 234.43256, 215.542, 230.19638, 213.2866, 218.26826, 205.42072, 212.00076, 205.17645, 203.56232, 203.94727, 193.56242, 187.9491, 178.99759, 173.63185, 162.99786, 167.54182, 154.81833, 149.77536, 153.43594, 135.09468, 132.44514, 126.85764, 126.54494, 118.79849, 108.33344, 103.64745, 100.90146, 86.41932, 70.56078, 77.56988, 70.58756, 64.53123, 59.12411, 43.693314, 39.51693, 31.62804, 17.614235, 5.442882, 7.2865133, -4.3905997, -16.295807, -20.42133, -31.24824, -30.792892, -39.684742, -47.08097, -51.443954, -63.032055, -82.773895, -80.921616, -85.259125, -87.84433, -107.72855, -115.419426, -117.800156, -129.57423, -129.15063, -133.22382, -142.07281, -151.42006, -149.80144, -151.13748, -166.01906, -164.31061, -175.02306, -182.56125, -183.112, -204.16766, -192.6448, -200.9696, -203.63722, -208.8648, -206.49487, -206.14053, -228.3682, -220.51105, -222.26875, -241.15546, -230.39905, -230.025, -235.60555, -225.78316, -235.51094, -237.73878, -230.10857, -229.67451, -231.38351, -234.38766, -222.30646, -226.3768, -232.44176, -228.48564, -236.51172, -224.73303, -228.71184, -222.64699, -222.5052, -212.23672, -219.0881, -209.59814, -209.15558, -210.46599, -199.85078, -207.3072, -196.99152, -202.2186, -192.57051, -178.88821, -177.45175, -177.78796, -152.55034, -166.74641, -153.75507, -146.85638, -147.27655, -140.6226, -132.4108, -135.81422, -125.47031, -122.31179, -102.785545, -101.163506, -92.88591, -84.36687, -72.38424, -75.31218, -64.309494, -51.889347, -46.02105, -37.522717, -35.8155, -24.43281, -22.818275, -21.093489, 4.9286413, 0.2512802, 15.619597, 21.425018, 24.468369, 30.323517, 44.334476, 48.330406, 71.46337, 68.28874, 79.5616, 78.860596, 89.62079, 103.98062, 101.84561, 112.053955, 118.05439, 122.465126, 130.91956, 140.62473, 143.17662, 149.55405, 158.19707, 168.31146, 173.37955, 174.15636, 188.19522, 179.25945, 177.89996, 200.6944, 194.04865, 188.76791, 203.79475, 213.96732, 215.90305, 209.42929, 202.8265, 225.78397, 220.42352, 224.89108, 231.52687, 241.48146, 234.32562, 238.60333, 237.6456, 232.71892, 240.64276, 234.70126, 236.51727, 236.01651, 235.97217, 237.10072, 233.68475, 231.95193, 228.87416, 225.9785, 227.46259, 218.48405, 226.39203, 210.50345, 222.48705, 213.98505, 212.96931, 209.06754, 202.2777, 202.58307, 197.74307, 193.59703, 192.5094, 180.30981, 183.31308, 174.39914, 161.19081, 160.79608, 155.41682, 149.26576, 134.91322, 153.52364, 134.63515, 124.065544, 127.12024, 111.52515, 108.357735, 97.63523, 88.24184, 82.07746, 79.3645, 74.673645, 61.02172, 50.545204, 53.34861, 51.895237, 22.94869, 36.04953, 4.5415926, 6.8501964, -9.68241, -3.3952348, -17.50255, -22.479744, -21.484806, -28.61837, -48.231236, -54.623753, -65.05635, -72.27062, -69.65976, -72.50991, -87.45172, -100.330795, -106.553375, -110.44685, -114.38192, -133.84885, -129.87274, -139.01674, -151.81104, -162.22218, -146.20099, -164.61877, -164.8809, -180.39383, -173.61903, -178.78201, -189.168, -188.9041, -193.93565, -198.47949, -213.20728, -214.42963, -212.68436, -207.04755, -224.92018, -222.3103, -220.3196, -234.41895, -235.49033, -227.22469, -222.27063, -226.01453, -232.94574, -233.54932, -232.33304, -226.25203, -240.39711, -226.14667, -222.75356, -231.45554, -227.59697, -229.28189, -237.97717, -232.8007, -243.1433, -226.78603, -228.60323, -233.67206, -207.89258, -211.41162, -212.8476, -205.51448, -194.04794, -196.3159, -187.42056, -194.55086, -184.6043, -182.27277, -175.28737, -162.52962, -165.55449, -161.45369, -147.52461, -143.47173, -132.15598, -145.62161, -128.15453, -114.47804, -115.03165, -114.793816, -113.90526, -85.86973, -93.94037, -80.591995, -69.852, -57.79867, -58.22773, -37.97185, -49.812187, -43.067924, -23.092434, -9.773935, -4.7970667, 1.3581278, -0.9040664, 14.689833, 26.247189, 39.266983, 28.56752, 34.871418, 49.339058, 58.06923, 68.292015, 62.994274, 86.75835, 96.49105, 89.816376, 86.03319, 114.309425, 112.405914, 113.22353, 122.32894, 129.3274, 136.81927, 143.05397, 148.1189, 151.28781, 162.25888, 160.39478, 174.34746, 178.38268, 185.59023, 193.31265, 183.7824, 198.43307, 204.33624, 210.62288, 210.95741, 219.86537, 212.19073, 212.7132, 222.94165, 227.31876, 230.47661, 230.49167, 232.18402, 231.2682, 220.42636, 235.34384, 237.90138, 241.80856, 229.12326, 234.13638, 235.93188, 224.63817, 231.22636, 225.19157, 221.73883, 224.78223, 228.44394, 233.02472, 218.71233, 227.30846, 218.15602, 210.87999, 210.56888, 201.95848, 201.70935, 206.59276, 195.87862, 199.99738, 186.69336, 188.11649, 181.54599, 174.82837, 172.8378, 158.61774, 153.56671, 158.43427, 152.32402, 145.50238, 135.41328, 129.54898, 114.0601, 113.32805, 104.36583, 97.06397, 87.11926, 87.36574, 70.94164, 71.11282, 69.87699, 49.80636, 53.929314, 39.71227, 34.022614, 21.744572, 17.192837, 18.630499, 13.065992, -10.085924, -7.667106, -18.49635, -20.80117, -34.73232, -46.397404, -56.461727, -50.291603, -69.4972, -74.70779, -75.74105, -78.843285, -83.81631, -107.750374, -99.66408, -112.136696, -135.6116, -129.35811, -134.18796, -144.52318, -140.77687, -148.45363, -158.15872, -156.91806, -171.88539, -175.83157, -178.65712, -181.25996, -186.22585, -185.19159, -198.51648, -196.64325, -193.73535, -205.78708, -218.49564, -206.64525, -211.20851, -223.60599, -227.45192, -232.10306, -229.47525, -225.05945, -227.95818, -231.98239, -243.06555, -222.94885, -238.6248, -236.3547, -223.28796, -230.99359, -227.7845, -235.14462, -241.14804, -228.95834, -221.64133, -217.4116, -219.40984, -225.07446, -221.46088, -214.94739, -210.73528, -216.32817, -204.11163, -191.5472, -210.3706, -200.24445, -180.9985, -187.33412, -191.9357, -182.2656, -177.02328, -162.77237, -154.49254, -160.13615, -143.06435, -133.17894, -148.99516, -120.932724, -134.616, -117.7417, -115.754875, -101.803535, -97.75104, -96.39932, -80.34772, -75.645645, -69.531204, -61.05463, -58.431015, -30.314415, -38.778824, -25.98773, -12.151533, -12.69001, -3.6732333, -4.6430845, 5.682135, 4.683598, 24.584915, 25.603477, 32.121464, 38.349712, 47.378674, 53.502, 75.00236, 68.05752, 78.07935, 77.238144, 93.845474, 101.03604, 113.18091, 128.16972, 129.54076, 125.866974, 133.32455, 142.00778, 142.56375, 147.01955, 152.82672, 162.6109, 168.11594, 167.37697, 181.67639, 191.77493, 184.25943, 197.97298, 203.44685, 204.46796, 203.5722, 222.88043, 210.18817, 210.80028, 207.08777, 221.68642, 222.81477, 213.49904, 227.3606, 237.51817, 239.3245, 232.8502, 246.0541, 240.06192, 237.26042, 222.49901, 233.31546, 244.29831, 234.2186, 232.25441, 235.10106, 229.36212, 236.46616, 225.54726, 225.93307, 221.33957, 217.3955, 219.73618, 209.30606, 211.8498, 195.95157, 198.69016, 196.61778, 197.9393, 183.06253, 179.4621, 178.77501, 170.59467, 165.6529, 162.2828, 147.95456, 156.78893, 136.54816, 137.10355, 140.99283, 135.02843, 122.19197, 115.060616, 102.78244, 97.978485, 86.40315, 87.95982, 89.0913, 63.21821, 64.91652, 61.774193, 65.27622, 53.093876, 41.077335, 35.62188, 25.559433, 21.312862, 6.2445383, 0.0058913045, -14.714803, -16.807858, -21.765642, -28.63797, -40.373333, -49.8555, -52.983597, -66.24956, -68.32419, -78.80607, -86.70257, -90.83329, -94.756836, -98.65308, -113.5187, -122.55146, -125.196846, -129.38293, -133.53853, -138.91887, -147.35692, -162.54262, -156.89404, -165.71873, -166.78598, -170.71918, -174.36105, -189.48756, -188.16942, -196.24532, -199.04536, -205.79948, -204.07285, -209.58585, -212.60733, -216.98929, -212.91849, -208.51164, -222.36534, -238.50359, -225.77548, -228.75032, -231.0378, -239.2212, -227.25781, -235.27614, -226.21664, -230.28639, -229.37651, -237.46422, -231.23468, -235.26125, -224.18387, -232.66742, -241.74957, -225.34094, -224.789, -225.57652, -221.34172, -225.14574, -202.9309, -214.37726, -204.16765, -196.31662, -201.50914, -191.2722, -198.09071, -179.1886, -170.96013, -175.39227, -157.99315, -160.36253, -155.25871, -147.56802, -141.18379, -137.71191, -135.02855, -130.3772, -137.1651, -100.227325, -107.639595, -94.45909, -89.32185, -86.86157, -66.011986, -63.815903, -62.614975, -54.89345, -42.768726, -34.171417, -30.411766, -30.05937, -23.441326, -8.866576, -6.361403, 13.222535, 5.051428, 20.283293, 20.52564, 42.396523, 49.830406, 45.304176, 55.49156, 57.52297, 71.534485, 87.43751, 82.9582, 93.69324, 90.415405, 106.038315, 116.017685, 124.93296, 137.38261, 132.27089, 138.5556, 138.03644, 156.77914, 142.323, 163.04843, 179.3619, 170.28006, 175.05305, 177.57977, 198.2261, 202.55058, 201.44583, 198.07545, 196.78644, 210.51643, 220.73639, 212.85316, 219.34308, 221.30174, 217.28734, 228.28703, 227.79716, 230.4997, 213.91928, 232.86772, 239.66142, 216.90884, 237.36673, 238.36667, 229.21178, 235.96077, 239.72556, 227.69234, 232.41254, 234.42493, 228.53795, 228.56071, 225.46034, 225.96225, 217.31924, 213.81836, 217.86124, 205.76537, 201.39555, 194.63948, 191.45735, 183.88463, 183.20627, 184.36342, 175.26717, 169.15742, 168.30942, 170.22209, 155.89848, 147.96304, 150.08044, 135.07033, 148.08522, 135.66692, 108.620544, 122.209854, 116.74914, 104.05033, 84.12573, 83.68529, 79.92133, 78.24319, 61.791515, 67.64047, 57.751556, 46.632923, 29.466003, 34.580578, 19.48428, 12.128019, -0.86505914, -7.2703495, -7.6162333, -16.399082, -29.126106, -28.468306, -42.700966, -56.35546, -62.04205, -74.39866, -61.30135, -77.66152, -83.61908, -88.99751, -102.52064, -98.31072, -110.24168, -118.48218, -124.33966, -132.10785, -130.62117, -144.12088, -147.91779, -152.35315, -165.13925, -167.5734, -167.13306, -176.03712, -173.30386, -194.41052, -192.17432, -192.9285, -200.58112, -204.08534, -208.81316, -204.77414, -208.67055, -217.37886, -223.06978, -225.96797, -231.79793, -228.85764, -228.94516, -223.35059, -220.35243, -227.38712, -242.84471, -225.80536, -232.54579, -230.02036, -234.04681, -225.29343, -225.16109, -232.52455, -225.62997, -238.81891, -229.65076, -220.36192, -228.19415, -217.80687, -215.42743, -224.78603, -210.788, -206.39165, -197.98257, -215.99747, -195.27989, -186.12497, -190.35173, -181.04477, -173.79309, -157.47295, -164.49542, -156.90134, -161.492, -141.49825, -144.99179, -129.67896, -128.78401, -132.94608, -117.39728, -108.1252, -106.32706, -101.02884, -80.61306, -94.47762, -78.81402, -70.11386, -55.58475, -48.774055, -51.194874, -35.29831, -33.416855, -22.210848, -14.76267, -7.388095, -9.17746, 9.691556, 23.218533, 36.10355, 22.366245, 39.687218, 46.01821, 67.253456, 56.294205, 56.575027, 69.19011, 87.94065, 81.58523, 106.020065, 105.23295, 111.989655, 119.64772, 134.49022, 142.13895, 123.8305, 143.4104, 138.5963, 156.8501, 158.55571, 170.13358, 166.27257, 168.64569, 182.92714, 185.05905, 192.67442, 200.32588, 193.77551, 203.69351, 212.2054, 204.45819, 214.31012, 214.2218, 213.99261, 223.99246, 233.12952, 237.75995, 232.25224, 231.26523, 247.62611, 232.70555, 235.17201, 234.62514, 235.59131, 233.694, 237.38374, 236.18091, 236.74336, 228.81802, 234.6565, 232.40932, 234.44514, 233.68117, 231.46577, 218.3994, 220.03574, 220.75798, 221.50758, 208.3501, 207.61922, 208.05777, 195.67972, 196.15186, 192.78226, 185.86725, 181.58649, 187.63866, 163.56866, 167.56892, 158.39569, 143.40256, 142.14476, 145.93939, 136.22691, 129.90222, 115.15274, 109.12108, 108.101494, 105.039055, 97.774345, 80.73653, 72.74583, 75.01072, 61.108753, 55.012527, 57.13765, 37.011173, 34.64829, 22.627771, 5.6822667, 11.878453, 1.5927191, -7.8100777, -10.215023, -6.2735763, -27.422718, -25.750729, -33.12553, -56.357662, -53.247944, -76.678116, -73.79516, -82.3833, -92.182465, -106.686775, -94.48443, -113.138954, -102.5368, -128.68591, -116.5446, -131.62857, -136.30965, -148.11072, -161.96469, -159.05205, -169.86429, -173.09944, -190.2189, -183.76889, -179.33456, -202.20338, -197.62222, -206.19437, -204.6209, -216.71083, -207.9178, -220.52577, -217.21906, -229.45476, -231.49973, -225.81165, -238.62614, -233.40588, -236.59991, -233.78442, -236.79744, -235.2981, -241.76256, -239.75064, -237.61412, -230.72606, -233.75056, -236.4871, -243.91202, -247.767, -231.95409, -228.66336, -220.48474, -225.40431, -227.82587, -219.78786, -219.67241, -209.0876, -212.73778, -213.09636, -207.51479, -206.75858, -190.20041, -196.06812, -189.22191, -201.14395, -186.81532, -179.9247, -169.02444, -152.87373, -156.22221, -147.40005, -145.65477, -144.43954, -134.32762, -124.819695, -109.20624, -111.74308, -99.38162, -107.312935, -98.318344, -85.4244, -76.41263, -76.816536, -52.078804, -49.557426, -47.941387, -38.792625, -35.484764, -13.184642, -8.305387, -12.917772, 1.9452688, 17.525309, 21.324387, 26.61016, 41.994125, 51.358032, 33.21182, 51.24739, 65.58397, 69.51333, 81.862785, 77.11882, 97.40104, 93.61309, 99.538445, 118.6689, 126.76111, 135.5323, 134.0534, 134.39285, 152.58429, 157.16483, 159.52333, 162.3537, 158.93327, 188.9048, 183.02353, 192.42851, 188.80818, 191.60226, 196.84346, 214.28995, 204.05649, 215.33653, 218.65442, 222.693, 218.38745, 221.2035, 235.56512, 235.34956, 253.00804, 236.85039, 228.57426, 234.28613, 247.82645, 243.39832, 248.1873, 238.844, 244.33882, 226.46469, 245.54094, 232.89937, 237.49448, 224.05121, 228.21573, 232.66277, 219.51826, 217.55386, 225.44182, 219.80147, 226.58609, 226.1954, 219.76135, 209.78618, 208.07701, 204.15225, 201.14102, 195.65466, 188.58032, 183.4892, 182.3676, 174.81943, 159.34633, 151.83762, 151.13223, 141.34576, 137.739, 127.62546, 122.75788, 123.067535, 107.04152, 110.78123, 102.743904, 108.52469, 89.29617, 76.26654, 66.45119, 65.4123, 68.241005, 56.423256, 49.176834, 35.39785, 19.903809, 22.087864, 4.751349, 4.5610967, -9.105463, -5.8854094, -8.188061, -22.59009, -40.405247, -51.71185, -55.786213, -56.49327, -72.978226, -65.8866, -94.83842, -101.17049, -105.12078, -103.25466, -120.27108, -116.03583, -121.07728, -121.28108, -132.1192, -144.68292, -154.83157, -154.79633, -168.30728, -165.59612, -184.57025, -189.42238, -197.35342, -182.64519, -194.32925, -207.85298, -221.6468, -212.85992, -221.93245, -227.80289, -214.60446, -224.45284, -236.49115, -224.71565, -251.57733, -229.04471, -235.05283, -254.29948, -240.80122, -251.0357, -245.77469, -240.60559, -246.1253, -239.44775, -239.8425, -236.6376, -250.01776, -237.87895, -235.99785, -247.43091, -243.27295, -236.33583, -235.83932, -227.89896, -231.92188, -225.38869, -217.47096, -199.69463, -211.77336, -207.09685, -214.13977, -217.59763, -204.07123, -201.60037, -192.94345, -181.24002, -169.81828, -170.1429, -163.35104, -161.57333, -156.62045, -139.51051, -143.57425, -128.26114, -128.69449, -125.75761, -105.516396, -100.968765, -98.28981, -82.77972, -86.987686, -80.482124, -62.05902, -63.191463, -43.177803, -47.35716, -20.289536, -19.233326, -27.315714, -10.527441, -2.0709991, 10.621492, 13.71096, 21.007744, 25.848375, 26.907877, 52.21863, 58.100258, 58.376205, 72.001366, 75.37558, 81.00366, 92.03348, 98.12794, 117.30527, 113.625, 133.18651, 126.41824, 130.74632, 138.2109, 146.03195, 154.3342, 169.95604, 162.221, 180.81787, 180.6959, 191.05153, 193.02736, 188.79388, 193.56886, 207.23201, 212.23611, 211.66275, 210.71425, 228.8026, 225.66415, 232.16727, 227.55215, 219.62006, 233.94705, 238.5536, 256.09457, 245.81978, 250.525, 255.38809, 255.01096, 247.00273, 257.48627, 258.6353, 237.82463, 248.62581, 249.98645, 249.09348, 253.15953, 253.05826, 238.4371, 239.9983, 245.72845, 235.8426], [-208.31999, -204.48, -200.16, -195.84, -191.28, -186.48, -181.44, -176.40001, -170.88, -165.36, -159.6, -153.59999, -147.6, -141.36, -134.87999, -128.40001, -121.68001, -114.96, -108.0, -100.799995, -93.6, -86.4, -78.96, -71.520004, -64.079994, -56.4, -48.719997, -41.04, -33.36, -25.44, -17.76, -9.84, -2.1599998, 5.76, 13.68, 21.36, 29.28, 36.96, 44.88, 52.559998, 60.0, 67.68, 75.119995, 82.560005, 90.0, 97.2, 104.159996, 111.36, 118.08, 124.799995, 131.51999, 138.0, 144.24, 150.48, 156.48, 162.48, 168.0, 173.52, 178.8, 183.84, 188.88, 193.44, 198.0, 202.31999, 206.40001, 210.23999, 213.84, 217.2, 220.31999, 223.2, 225.84, 228.23999, 230.4, 232.31999, 234.0, 235.44, 236.64, 237.6, 238.08, 238.56, 238.8, 238.56, 238.08, 237.6, 236.64, 235.44, 234.0, 232.31999, 230.4, 228.23999, 225.84, 223.2, 220.31999, 217.2, 213.84, 210.23999, 206.40001, 202.31999, 198.0, 193.68, 188.88, 184.08, 178.8, 173.52, 168.23999, 162.48, 156.72, 150.72, 144.48, 138.23999, 131.76001, 125.04001, 118.32, 111.36, 104.4, 97.2, 90.0, 82.8, 75.36, 67.92, 60.239998, 52.559998, 44.88, 37.2, 29.52, 21.6, 13.92, 6.0, -1.9200001, -9.84, -17.52, -25.44, -33.12, -41.04, -48.719997, -56.4, -63.84, -71.520004, -78.96, -86.159996, -93.6, -100.799995, -107.76, -114.71999, -121.439995, -128.15999, -134.87999, -141.12, -147.36, -153.59999, -159.36, -165.12001, -170.88, -176.16, -181.44, -186.48, -191.28, -195.84, -200.16, -204.24, -208.31999, -211.92, -215.52, -218.88, -221.76001, -224.64, -227.04, -229.43999, -231.36, -233.28, -234.72, -236.16, -237.12, -237.84, -238.31999, -238.56, -238.56, -238.31999, -237.84, -237.12, -236.16, -234.72, -233.28, -231.59999, -229.43999, -227.04, -224.64, -221.76001, -218.88, -215.52, -212.16, -208.31999, -204.48, -200.16, -195.84, -191.28, -186.48, -181.44, -176.40001, -170.88, -165.36, -159.6, -153.59999, -147.6, -141.36, -134.87999, -128.40001, -121.68001, -114.71999, -108.0, -100.799995, -93.6, -86.4, -78.96, -71.520004, -64.079994, -56.4, -48.719997, -41.04, -33.36, -25.44, -17.76, -9.84, -1.9200001, 5.76, 13.68, 21.6, 29.28, 37.2, 44.88, 52.559998, 60.239998, 67.68, 75.119995, 82.560005, 90.0, 97.2, 104.4, 111.36, 118.08, 125.04001, 131.51999, 138.0, 144.48, 150.48, 156.48, 162.48, 168.0, 173.52, 178.8, 183.84, 188.88, 193.44, 198.0, 202.31999, 206.40001, 210.23999, 213.84, 217.2, 220.31999, 223.2, 225.84, 228.23999, 230.4, 232.31999, 234.0, 235.44, 236.64, 237.6, 238.08, 238.56, 238.8, 238.56, 238.08, 237.6, 236.64, 235.44, 234.0, 232.31999, 230.4, 228.23999, 225.84, 223.2, 220.31999, 217.2, 213.84, 210.23999, 206.40001, 202.31999, 198.0, 193.68, 188.88, 184.08, 178.8, 173.52, 168.0, 162.48, 156.72, 150.72, 144.48, 138.0, 131.51999, 125.04001, 118.32, 111.36, 104.4, 97.2, 90.0, 82.8, 75.36, 67.68, 60.239998, 52.559998, 44.88, 37.2, 29.52, 21.6, 13.68, 6.0, -1.9200001, -9.84, -17.52, -25.44, -33.12, -41.04, -48.719997, -56.4, -63.84, -71.520004, -78.96, -86.4, -93.6, -100.799995, -107.76, -114.71999, -121.68001, -128.15999, -134.87999, -141.12, -147.6, -153.59999, -159.6, -165.36, -170.88, -176.16, -181.44, -186.48, -191.28, -195.84, -200.16, -204.48, -208.31999, -212.16, -215.52, -218.88, -221.76001, -224.64, -227.04, -229.43999, -231.36, -233.28, -234.72, -236.16, -237.12, -237.84, -238.31999, -238.56, -238.56, -238.31999, -237.84, -237.12, -236.16, -234.72, -233.28, -231.36, -229.43999, -227.04, -224.64, -221.76001, -218.88, -215.52, -212.16, -208.31999, -204.48, -200.16, -195.84, -191.28, -186.48, -181.44, -176.16, -170.88, -165.36, -159.6, -153.59999, -147.6, -141.36, -134.87999, -128.40001, -121.68001, -114.71999, -107.76, -100.799995, -93.6, -86.4, -78.96, -71.520004, -64.079994, -56.4, -48.719997, -41.04, -33.36, -25.44, -17.76, -9.84, -1.9200001, 5.76, 13.68, 21.6, 29.28, 37.2, 44.88, 52.559998, 60.239998, 67.68, 75.119995, 82.560005, 90.0, 97.2, 104.4, 111.36, 118.32, 125.04001, 131.51999, 138.0, 144.48, 150.48, 156.48, 162.48, 168.0, 173.52, 178.8, 184.08, 188.88, 193.68, 198.0, 202.31999, 206.40001, 210.23999, 213.84, 217.2, 220.31999, 223.2, 225.84, 228.23999, 230.4, 232.31999, 234.0, 235.44, 236.64, 237.6, 238.08, 238.56, 238.8, 238.56, 238.08, 237.6, 236.64, 235.44, 234.0, 232.31999, 230.4, 228.23999, 225.84, 223.2, 220.31999, 217.2, 213.84, 210.23999, 206.40001, 202.31999, 198.0, 193.68, 188.88, 184.08, 178.8, 173.52, 168.0, 162.48, 156.48, 150.48, 144.48, 138.0, 131.51999, 125.04001, 118.32, 111.36, 104.4, 97.2, 90.0, 82.560005, 75.36, 67.68, 60.239998, 52.559998, 44.88, 37.2, 29.28, 21.6, 13.68, 6.0, -1.9200001, -9.84, -17.76, -25.44, -33.36, -41.04, -48.719997, -56.4, -64.079994, -71.520004, -78.96, -86.4, -93.6, -100.799995, -107.76, -114.71999, -121.68001, -128.40001, -134.87999, -141.36, -147.6, -153.59999, -159.6, -165.36, -170.88, -176.16, -181.44, -186.48, -191.28, -195.84, -200.16, -204.48, -208.31999, -212.16, -215.52, -218.88, -221.76001, -224.64, -227.04, -229.43999, -231.36, -233.28, -234.72, -236.16, -237.12, -237.84, -238.31999, -238.56, -238.56, -238.31999, -237.84, -237.12, -236.16, -234.72, -233.28, -231.36, -229.43999, -227.04, -224.64, -221.76001, -218.88, -215.52, -212.16, -208.31999, -204.48, -200.16, -195.84, -191.28, -186.48, -181.44, -176.16, -170.88, -165.36, -159.6, -153.59999, -147.6, -141.36, -134.87999, -128.40001, -121.68001, -114.71999, -107.76, -100.799995, -93.6, -86.4, -78.96, -71.520004, -64.079994, -56.4, -48.719997, -41.04, -33.36, -25.44, -17.52, -9.84, -1.9200001, 6.0, 13.68, 21.6, 29.28, 37.2, 44.88, 52.559998, 60.239998, 67.68, 75.36, 82.8, 90.0, 97.2, 104.4, 111.36, 118.32, 125.04001, 131.51999, 138.0, 144.48, 150.48, 156.72, 162.48, 168.0, 173.52, 178.8, 184.08, 188.88, 193.68, 198.0, 202.31999, 206.40001, 210.23999, 213.84, 217.2, 220.31999, 223.2, 225.84, 228.23999, 230.4, 232.31999, 234.0, 235.44, 236.64, 237.6, 238.08, 238.56, 238.8, 238.56, 238.08, 237.6, 236.64, 235.44, 234.0, 232.31999, 230.4, 228.23999, 225.84, 223.2, 220.31999, 217.2, 213.84, 210.23999, 206.40001, 202.31999, 198.0, 193.44, 188.88, 183.84, 178.8, 173.52, 168.0, 162.48, 156.48, 150.48, 144.48, 138.0, 131.51999, 125.04001, 118.08, 111.36, 104.4, 97.2, 90.0, 82.560005, 75.119995, 67.68, 60.239998, 52.559998, 44.88, 37.2, 29.28, 21.6, 13.68, 5.76, -1.9200001, -9.84, -17.76, -25.44, -33.36, -41.04, -48.719997, -56.4, -64.079994, -71.520004, -78.96, -86.4, -93.6, -100.799995, -107.76, -114.71999, -121.68001, -128.40001, -134.87999, -141.36, -147.6, -153.59999, -159.6, -165.36, -170.88, -176.16, -181.44, -186.48, -191.28, -195.84, -200.16, -204.48, -208.31999, -212.16, -215.52, -218.88, -221.76001, -224.64, -227.04, -229.43999, -231.59999, -233.28, -234.72, -236.16, -237.12, -237.84, -238.31999, -238.56, -238.56, -238.31999, -237.84, -237.12, -236.16, -234.72, -233.28, -231.36, -229.43999, -227.04, -224.64, -221.76001, -218.88, -215.52, -211.92, -208.31999, -204.48, -200.16, -195.84, -191.28, -186.48, -181.44, -176.16, -170.88, -165.36, -159.6, -153.59999, -147.36, -141.12, -134.87999, -128.15999, -121.68001, -114.71999, -107.76, -100.799995, -93.6, -86.4, -78.96, -71.520004, -63.84, -56.4, -48.719997, -41.04, -33.12, -25.44, -17.52, -9.84, -1.9200001, 6.0, 13.68, 21.6, 29.52, 37.2, 44.88, 52.559998, 60.239998, 67.92, 75.36, 82.8, 90.0, 97.2, 104.4, 111.36, 118.32, 125.04001, 131.51999, 138.0, 144.48, 150.72, 156.72, 162.48, 168.23999, 173.52, 178.8, 184.08, 188.88, 193.68, 198.0, 202.31999, 206.40001, 210.23999, 213.84, 217.2, 220.31999, 223.2, 225.84, 228.23999, 230.4, 232.31999, 234.0, 235.44, 236.64, 237.6, 238.08, 238.56, 238.8, 238.56, 238.08, 237.6, 236.64, 235.44, 234.0, 232.31999, 230.4, 228.23999, 225.84, 223.2, 220.31999, 217.2, 213.84, 210.23999, 206.40001, 202.31999, 198.0, 193.44, 188.88, 183.84, 178.8, 173.52, 168.0, 162.48, 156.48, 150.48, 144.24, 138.0, 131.51999, 124.799995, 118.08, 111.36, 104.159996, 97.2, 90.0, 82.560005, 75.119995, 67.68, 60.239998, 52.559998, 44.88, 36.96, 29.28, 21.6, 13.68, 5.76, -1.9200001, -9.84, -17.76, -25.44, -33.36, -41.04, -48.719997, -56.4, -64.079994, -71.520004, -78.96, -86.4, -93.6, -100.799995, -108.0, -114.96, -121.68001, -128.40001, -134.87999, -141.36, -147.6, -153.59999, -159.6, -165.36, -170.88, -176.40001, -181.44, -186.48, -191.28, -195.84, -200.16, -204.48, -208.31999, -212.16, -215.52, -218.88, -221.76001, -224.64, -227.28, -229.43999, -231.59999, -233.28, -234.72, -236.16, -237.12, -237.84, -238.31999, -238.56, -238.56, -238.31999, -237.84, -237.12, -236.16, -234.72, -233.28, -231.36, -229.43999, -227.04, -224.64, -221.76001, -218.88, -215.52, -211.92, -208.31999, -204.24, -298.56, -291.84, -285.12, -277.91998, -270.47998, -262.80002, -254.64, -246.47998, -237.84, -228.95999, -219.84, -210.48, -200.88, -191.28, -181.2, -171.12, -160.8, -150.23999, -139.43999, -128.64, -117.600006, -106.56, -95.28001, -84.0, -72.479996, -60.960003, -49.44, -37.920002, -26.16, -14.4, -2.88, 8.88, 20.640001, 32.4, 43.92, 55.440002, 66.96001, 78.479996, 90.0, 101.28, 112.32, 123.36, 134.4, 144.95999, 155.76, 166.07999, 176.40001, 186.48, 196.32, 205.92, 215.52, 224.64, 233.52, 242.4, 250.79999, 258.96, 266.88, 274.32, 281.76, 288.72, 295.44, 301.68, 307.91998, 313.44, 318.96, 324.0, 328.56, 332.88, 336.96002, 340.56, 343.68002, 346.56, 348.96, 351.12003, 352.80002, 354.24, 355.2, 355.68, 355.92, 355.68, 355.2, 354.24, 352.80002, 351.12003, 348.96, 346.56, 343.68002, 340.32, 336.72, 332.88, 328.56, 323.76, 318.72, 313.44, 307.68, 301.68, 295.2, 288.48, 281.52, 274.32, 266.63998, 258.72, 250.56001, 242.15999, 233.28, 224.4, 215.28, 205.68, 196.07999, 186.24, 176.16, 165.84, 155.52, 144.72, 133.92001, 123.12, 112.08, 100.799995, 89.52, 78.24, 66.72, 55.2, 43.68, 31.92, 20.4, 8.639999, -3.1200001, -14.88, -26.4, -38.16, -49.68, -61.440002, -72.72, -84.240005, -95.520004, -106.799995, -117.84, -128.88, -139.68001, -150.48, -161.04001, -171.36, -181.44, -191.51999, -201.12, -210.72, -220.08, -229.2, -238.08, -246.47998, -254.88, -262.80002, -270.72, -278.16, -285.36002, -292.08002, -298.56, -304.8, -310.8, -316.31998, -321.36, -326.4, -330.72, -335.04, -338.64, -342.24, -345.12, -347.76, -350.16, -352.08002, -353.52002, -354.72, -355.44, -355.92, -355.92, -355.44, -354.72, -353.52002, -352.08002, -350.16, -347.76, -345.12, -342.0, -338.64, -334.8, -330.72, -326.16, -321.36, -316.08002, -310.56, -304.8, -298.56, -291.84, -285.12, -277.91998, -270.47998, -262.80002, -254.64, -246.24, -237.84, -228.95999, -219.84, -210.48, -200.88, -191.04001, -181.2, -171.12, -160.56001, -150.0, -139.43999, -128.64, -117.600006, -106.56, -95.28001, -84.0, -72.479996, -60.960003, -49.44, -37.68, -26.16, -14.4, -2.6399999, 8.88, 20.640001, 32.4, 43.92, 55.68, 67.2, 78.479996, 90.0, 101.28, 112.32, 123.36, 134.4, 145.20001, 155.76, 166.07999, 176.40001, 186.48, 196.32, 205.92, 215.52, 224.64, 233.52, 242.4, 250.79999, 258.96, 266.88, 274.56, 281.76, 288.72, 295.44, 301.92, 307.91998, 313.68002, 318.96, 324.0, 328.56, 332.88, 336.96002, 340.56, 343.68002, 346.56, 348.96, 351.12003, 352.80002, 354.24, 355.2, 355.68, 355.92, 355.68, 355.2, 354.24, 352.80002, 351.12003, 348.96, 346.56, 343.68002, 340.32, 336.72, 332.88, 328.56, 323.76, 318.72, 313.44, 307.68, 301.68, 295.2, 288.48, 281.52, 274.08, 266.63998, 258.72, 250.56001, 242.15999, 233.28, 224.4, 215.04001, 205.68, 196.07999, 186.24, 176.16, 165.84, 155.28, 144.72, 133.92001, 123.12, 112.08, 100.799995, 89.52, 78.24, 66.72, 55.2, 43.68, 31.92, 20.16, 8.639999, -3.1200001, -14.88, -26.64, -38.16, -49.920002, -61.440002, -72.96, -84.240005, -95.520004, -106.799995, -117.84, -128.88, -139.68001, -150.48, -161.04001, -171.36, -181.44, -191.51999, -201.36, -210.72, -220.08, -229.2, -238.08, -246.72, -254.88, -263.03998, -270.72, -278.16, -285.36002, -292.08002, -298.8, -304.8, -310.8, -316.31998, -321.6, -326.4, -330.96, -335.04, -338.64, -342.24, -345.12, -347.76, -350.16, -352.08002, -353.52002, -354.72, -355.44, -355.92, -355.92, -355.44, -354.72, -353.52002, -352.08002, -350.16, -347.76, -345.12, -342.0, -338.64, -334.8, -330.72, -326.16, -321.36, -316.08002, -310.56, -304.56, -298.32, -291.84, -285.12, -277.91998, -270.47998, -262.56, -254.64, -246.24, -237.6, -228.95999, -219.84, -210.48, -200.88, -191.04001, -181.2, -170.88, -160.56001, -150.0, -139.43999, -128.40001, -117.600006, -106.32, -95.28001, -83.76, -72.479996, -60.960003, -49.44, -37.68, -26.16, -14.4, -2.6399999, 9.12, 20.640001, 32.4, 43.92, 55.68, 67.2, 78.72, 90.0, 101.28, 112.560005, 123.6, 134.4, 145.20001, 155.76, 166.32, 176.40001, 186.48, 196.32, 206.16, 215.52, 224.64, 233.76, 242.4, 250.79999, 258.96, 266.88, 274.56, 281.76, 288.72, 295.44, 301.92, 307.91998, 313.68002, 318.96, 324.0, 328.56, 332.88, 336.96002, 340.56, 343.68002, 346.56, 348.96, 351.12003, 352.80002, 354.24, 238.08, 238.56, 238.8, 238.56, 238.08, 237.6, 236.64, 235.44, 234.0, 232.31999, 230.4, 228.23999, 225.84, 223.2, 220.31999, 217.2, 213.84, 210.23999, 206.40001, 202.31999, 198.0, 193.44, 188.88, 183.84, 178.8, 173.52, 168.0, 162.24, 156.48, 150.48, 144.24, 138.0, 131.51999, 124.799995, 118.08, 111.12, 104.159996, 96.96001, 89.76, 82.560005, 75.119995, 67.68, 60.0, 52.32, 44.64, 36.96, 29.28, 21.36, 13.440001, 5.76, -2.1599998, -10.08, -17.76, -25.68, -33.36, -41.280003, -48.96, -56.64, -64.079994, -71.76, -79.200005, -86.4, -93.840004, -101.04, -108.0, -114.96, -121.68001, -128.40001, -134.87999, -141.36, -147.6, -153.84, -159.6, -165.36, -170.88, -176.40001, -181.68001, -186.48, -191.28, -195.84, -200.4, -204.48, -208.31999, -212.16, -215.52, -218.88, -222.0, -224.64, -227.28, -229.43999, -231.59999, -233.28, -234.72, -236.16, -237.12, -237.84, -238.31999, -238.56, -238.56, -238.31999, -237.84, -237.12, -236.16, -234.72, -233.28, -231.36, -229.43999, -227.04, -224.64, -221.76001, -218.64, -215.52, -211.92, -208.31999, -204.24, -200.16, -195.84, -191.04001, -186.24, -181.44, -176.16, -170.64, -165.12001, -159.36, -153.36, -147.36, -141.12, -134.64, -128.15999, -121.439995, -114.71999, -107.76, -100.56, -93.36, -86.159996, -78.72, -71.28, -63.84, -56.16, -48.480003, -40.8, -33.12, -25.199999, -17.52, -9.599999, -1.6800001, 6.0, 13.92, 21.84, 29.52, 37.440002, 45.12, 52.8, 60.48, 67.92, 75.36, 82.8, 90.24, 97.439995, 104.4, 111.6, 118.32, 125.04001, 131.76001, 138.23999, 144.48, 150.72, 156.72, 162.48, 168.23999, 173.76, 179.04, 184.08, 188.88, 193.68, 198.23999, 202.56, 206.40001, 210.23999, 213.84, 217.2, 220.31999, 223.2, 226.07999, 228.48001, 230.64, 232.56, 234.0, 235.44, 236.64, 237.6, 238.08, 238.56, 238.8, 238.56, 238.08, 237.6, 236.64, 235.44, 234.0, 232.31999, 230.4, 228.23999, 225.84, 223.2, 220.31999, 217.2, 213.84, 210.23999, 206.40001, 202.31999, 198.0, 193.44, 188.64, 183.84, 178.8, 173.52, 168.0, 162.24, 156.48, 150.48, 144.24, 138.0, 131.51999, 124.799995, 118.08, 111.12, 104.159996, 96.96001, 89.76, 82.560005, 75.119995, 67.439995, 60.0, 52.32, 44.64, 36.96, 29.28, 21.36, 13.440001, 5.76, -2.1599998, -10.08, -17.76, -25.68, -33.36, -41.280003, -48.96, -56.64, -64.079994, -71.76, -79.200005, -86.64, -93.840004, -101.04, -108.0, -114.96, -121.68001, -128.40001, -135.12001, -141.36, -147.6, -153.84, -159.6, -165.36, -171.12, -176.40001, -181.68001, -186.48, -191.28, -196.07999, -200.4, -204.48, -208.56, -212.16, -215.52, -218.88, -222.0, -224.64, -227.28, -229.43999, -231.59999, -233.28, -234.95999, -236.16, -237.12, -237.84, -238.31999, -238.56, -238.56, -238.31999, -237.84, -237.12, -236.16, -234.72, -233.28, -231.36, -229.43999, -227.04, -224.64, -221.76001, -218.64, -215.52, -211.92, -208.31999, -204.24, -200.16, -195.6, -191.04001, -186.24, -181.2, -176.16, -170.64, -165.12001, -159.36, -153.36, -147.36, -141.12, -134.64, -128.15999, -121.439995, -114.479996, -107.520004, -100.56, -93.36, -86.159996, -78.72, -71.28, -63.84, -56.16, -48.480003, -40.8, -33.12, -25.199999, -17.52, -9.599999, -1.6800001, 6.0, 13.92, 21.84, 29.52, 37.440002, 45.12, 52.8, 60.48, 67.92, 75.36, 82.8, 90.24, 97.439995, 104.64, 111.6, 118.32, 125.28001, 131.76001, 138.23999, 144.48, 150.72, 156.72, 162.48, 168.23999, 173.76, 179.04, 184.08, 189.12, 193.68, 198.23999, 202.56, 206.40001, 210.23999, 213.84, 217.2, 220.31999, 223.44, 226.07999, 228.48001, 230.64, 232.56, 234.0, 235.44, 236.64, 237.6, 238.08, 238.56, 238.8, 238.56, 238.08, 237.6, 236.64, 235.44, 234.0, 232.31999, 230.4, 228.23999, 225.84, 223.2, 220.31999, 217.2, 213.84, 210.0, 206.16, 202.31999, 198.0, 193.44, 188.64, 183.84, 178.8, 173.52, 168.0, 162.24, 156.48, 150.48, 144.24, 137.76, 131.28, 124.799995, 118.08, 111.12, 104.159996, 96.96001, 89.76, 82.32, 75.119995, 67.439995, 60.0, 52.32, 44.64, 36.96, 29.039999, 21.36, 13.440001, 5.76, -2.1599998, -10.08, -18.0, -25.68, -33.6, -41.280003, -48.96, -56.64, -64.32, -71.76, -79.200005, -86.64, -93.840004, -101.04, -108.0, -114.96, -121.920006, -128.40001, -135.12001, -141.36, -147.6, -153.84, -159.6, -165.36, -171.12, -176.40001, -181.68001, -186.72, -191.51999, -196.07999, -200.4, -204.48, -208.56, -212.16, -215.76, -218.88, -222.0, -224.64, -227.28, -229.43999, -231.59999, -233.28, -234.95999, -236.16, -237.12, -237.84, -238.31999, -238.56, -238.56, -238.31999, -237.84, -237.12, -236.16, -234.72, -233.28, -231.36, -229.43999, -227.04, -224.4, -221.76001, -218.64, -215.52, -211.92, -208.31999, -204.24, -200.16, -195.6, -191.04001, -186.24, -181.2, -176.16, -170.64, -165.12001, -159.36, -153.36, -147.36, -141.12, -134.64, -128.15999, -121.439995, -114.479996, -107.520004, -100.56, -93.36, -86.159996, -78.72, -71.28, -63.84, -56.16, -48.480003, -40.8, -33.12, -25.199999, -17.279999, -9.599999, -1.6800001, 6.2400002, 13.92, 21.84, 29.52, 37.440002, 45.12, 52.8, 60.48, 67.92, 75.6, 82.8, 90.24, 97.439995, 104.64, 111.6, 118.56, 125.28001, 131.76001, 138.23999, 144.72, 150.72, 156.72, 162.72, 168.23999, 173.76, 179.04, 184.08, 189.12, 193.68, 198.23999, 202.56, 206.64, 210.23999, 213.84, 217.2, 220.56001, 223.44, 226.07999, 228.48001, 230.64, 232.56, 234.0, 235.44, 236.64, 237.6, 238.31999, 238.56, 238.8, 238.56, 238.08, 237.6, 236.64, 235.44, 234.0, 232.31999, 230.4, 228.23999]]
  in  "Stop":bool
  in  "Sample Index":i32=318 min=0 max=499
  in  "Check?":bool
  out "Train Speed (Samples/sec)":dbl=16812.228164006938 format="%_3p"
  out "Train Speed (sec/iter)":dbl=0.00761350599999787 format="%_3p"
  out "Train Loss":sgl=5.3138003 format="%.3g"
  out "Time_Elapsed":dbl=22.13641259999895 format="%<%H:%M:%S>t"
  out "Session Data":T1={"Epochs"=32.832, "Tot_Iter"=2565, "LR"=1.25e-05, "LR_iter"=2566}
  in  "LR Update Policy":T2={"Policy_Type"=enum."Step", "LR0"=0.0001, "k"=10.0, "WarmUp_Policy"=enum."Ramp", "WarmUp_Iter"=600, "WarmUp_Ratio"=20.0} {"WarmUp_Ratio" min=1; "WarmUp_Iter" min=1; "LR0" format="%.7f"}
  in  "Train_Params":T4={"Optimizer"=enum."Adam", "Beta_1"=0.9, "Beta_2"=0.999, "Weight Decay(L1)"=0.0, "Weight Decay(L2)"=0.0, "Data_Sampling"=enum."Random"}
  in  "NN_Device":T7=enum."GPU"
  # "Overview: This example demonstrates how to use DeepLTK to perform anomaly detection on power line data using an autoencoder-based architecture.\nRequirments: Deep Learning Toolkit for LabVIEW.\nInstructions:\n1. Provide Train and Validation (Normal/Abnormal) dataset paths.\n2. Run the VI using the default configuration settings.\n3. Observe how the training loss is decreasing. Observe the training speed.\n4. Periodically press the \"Eval\" button to evaluate the autoencoder's performance on both normal and abnormal validation samples.\n5. Wait until the loss curve reaches its minimum. Approximately 30 epochs.\n6. Stop the VI.\n7. Open the file \"2_WF_Anomaly_Detection(Threshold_Evaluation).vi\" to evaluate the anomaly detection threshold."
  # "Waveform Anomaly Detection - Training"
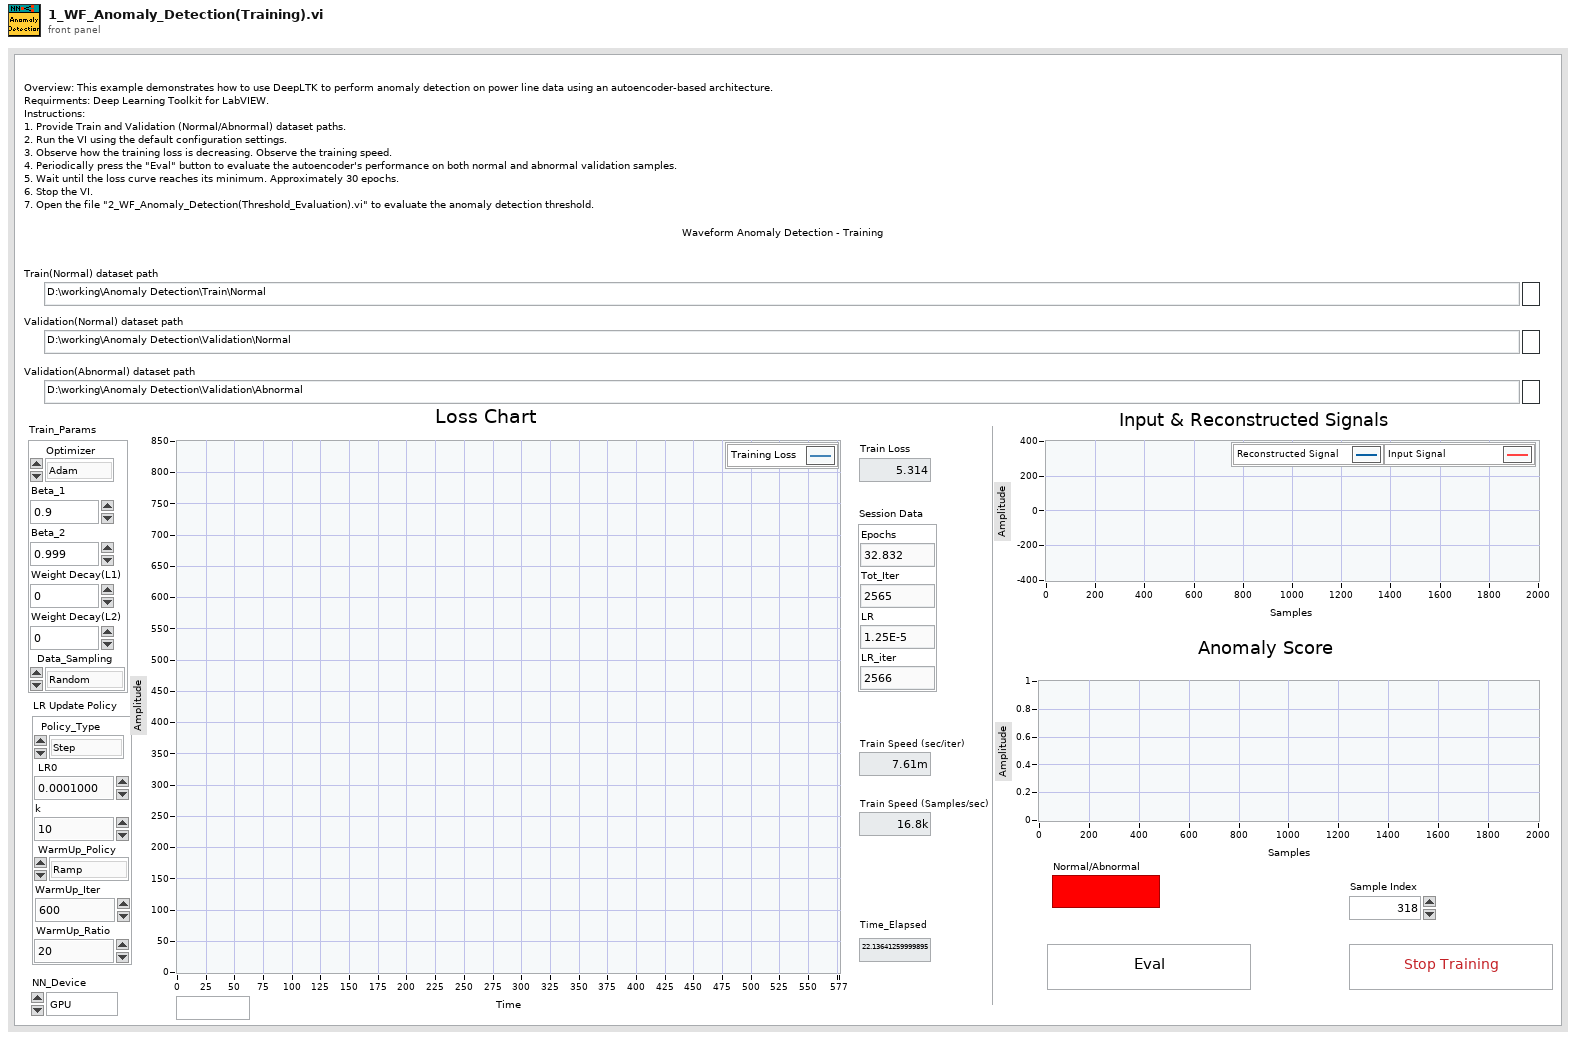
[diagram p1: front panel]
types:
  T1 = typedef "Deep_Learning_Toolkit_by_Ngene.lvlib/NN_Train_Session_Data.ctl" = cluster{"Epochs":sgl, "Tot_Iter":i32, "LR":sgl, "LR_iter":i32}
  T2 = typedef "Deep_Learning_Toolkit_by_Ngene.lvlib/NN_LR_Policy_Cfg.ctl" = cluster{"Policy_Type":T3, "LR0":dbl, "k":sgl, "WarmUp_Policy":enum16{"Step", "Ramp"}, "WarmUp_Iter":i32, "WarmUp_Ratio":sgl}
  T3 = typedef "Deep_Learning_Toolkit_by_Ngene.lvlib/NN_LR_Policy_Type.ctl" = enum16{"Manual", "Step", "Exp", "1/t"}
  T4 = typedef "Deep_Learning_Toolkit_by_Ngene.lvlib/NN_Train_Params.ctl" = cluster{"Optimizer":T5, "Beta_1":sgl, "Beta_2":sgl, "Weight Decay(L1)":sgl, "Weight Decay(L2)":sgl, "Data_Sampling":T6}
  T5 = typedef "Deep_Learning_Toolkit_by_Ngene.lvlib/NN_Train_Optimizer.ctl" = enum16{"SGD", "Adam", "Adagrad", "Adadelta", "RMSProp", "Nesterov"}
  T6 = typedef "Deep_Learning_Toolkit_by_Ngene.lvlib/NN_Train_Data_Sampling.ctl" = enum16{"Random", "Sequential"}
  T7 = typedef "Deep_Learning_Toolkit_by_Ngene.lvlib/NN_Device.ctl" = enum16{"CPU", "GPU"}
  T8 = typedef "Deep_Learning_Toolkit_by_Ngene.lvlib/NN_Layer_Config_Aug(Input1D).ctl" = T9[]
  T9 = typedef "Deep_Learning_Toolkit_by_Ngene.lvlib/NN_Input1D_Aug_Config.ctl" = cluster{"Aug Type(1D)":T10, "Aug Value":sgl, "Distribution":T11}
  T10 = typedef "Deep_Learning_Toolkit_by_Ngene.lvlib/NN_Input1D_Aug_Types.ctl" = enum16{"Add_Noise", "Mult_Noise", "Shift", "Scale"}
  T11 = typedef "Deep_Learning_Toolkit_by_Ngene.lvlib/Aug_Distribution_Type.ctl" = enum16{"Uniform", "Gaussian"}
  T12 = typedef "Deep_Learning_Toolkit_by_Ngene.lvlib/NN_Layer_Config(FC).ctl" = cluster{"Name":string, "Size":i32, "BN":bool, "BN_Params":T13, "Activation":T14, "Has Bias?":bool, "Init_Params":T15, "Custom_Params":string}
  T13 = typedef "Deep_Learning_Toolkit_by_Ngene.lvlib/NN_BN_Params.ctl" = cluster{"epsilon":sgl, "momentum":sgl}
  T14 = typedef "Deep_Learning_Toolkit_by_Ngene.lvlib/NN_Activation_Type.ctl" = enum16{"Sigmoid", "ReLU", "LReLU", "ReLU6", "GELU", "tanh", "Swish", "Mish", "None"}
  T15 = typedef "Deep_Learning_Toolkit_by_Ngene.lvlib/NN_Layer_Init_Params.ctl" = cluster{"Init_Type":T16, "Value":sgl}
  T16 = typedef "Deep_Learning_Toolkit_by_Ngene.lvlib/NN_Layer_Weight_Init_Type.ctl" = enum16{"Const", "Uniform", "Gaussian", "Xavier"}
  T17 = typedef "Deep_Learning_Toolkit_by_Ngene.lvlib/NN_Layer_Config(Input1D).ctl" = cluster{"Name":string, "Size":i32, "Data_Type":T18, "Shift":sgl, "Scale":sgl}
  T18 = typedef "Deep_Learning_Toolkit_by_Ngene.lvlib/NN_Data_type.ctl" = enum16{"I8", "U8", "I16", "U16", "U32 ARGB", "SGL"}
  T19 = typedef "Deep_Learning_Toolkit_by_Ngene.lvlib/NN_Save_Before_Destroy_Options.ctl" = cluster{"CFG?":bool, "Weights?":bool, "Render?":bool}
  T20 = typedef "Deep_Learning_Toolkit_by_Ngene.lvlib/NN_DataSet(In1D_Out1D).ctl" = cluster{"Inputs Ref.":variant, "Outputs Ref.":T21, "Dims_In":i32, "Dataset_Size":i32, "Dims_Out":i32, "Labels":string[], "File Paths":path[], "Custom_Data":variant}
  T21 = typedef "Deep_Learning_Toolkit_by_Ngene.lvlib/NN_Data_ref(2D_SGL).ctl" = refnum<data-value>
  T22 = typedef "Deep_Learning_Toolkit_by_Ngene.lvlib/NN.ctl" = cluster{"Name":string, "No of Layers":i32, "mBatch":i32, "Layers":T23[], "Dimty":T24, "Dims_In":T25, "Dims_Out":T25, "Working_Dir":path, "Train?":bool, "Train_Params":T4, "LR_Update_Policy":T2, "Session Data":T1, "Ground_truth":T26, "NNg_hdls":T27, "NN_Device":T7, "GPU Id":i32, "Labels":string[], "Loss_Type":T28, "Loss_Cfg_Prms":variant, "NNG_WS":T29, "DryRun?":bool}
  T23 = typedef "Deep_Learning_Toolkit_by_Ngene.lvlib/NN_Layer_ref.ctl" = refnum<file>
  T24 = typedef "Deep_Learning_Toolkit_by_Ngene.lvlib/NN_In_Out_Dim-ty.ctl" = enum8{"In1D_Out1D", "In3D_Out1D", "In3D_Out3D", "In3D_OutBBox"}
  T25 = typedef "Deep_Learning_Toolkit_by_Ngene.lvlib/NN_Dims(C,H,W).ctl" = cluster{"C":i32, "H":i32, "W":i32}
  T26 = typedef "Deep_Learning_Toolkit_by_Ngene.lvlib/NN_Ground_truth.ctl" = cluster{"Y":variant}
  T27 = typedef "Deep_Learning_Toolkit_by_Ngene.lvlib/nng_cuda_handles.ctl" = cluster{"cudnn":u64, "cublas":u64, "stream":u64, "curand":u64}
  T28 = typedef "Deep_Learning_Toolkit_by_Ngene.lvlib/NN_Loss_Type.ctl" = enum16{"None", "MSE", "CrossEntropy", "YOLO_v2", "YOLO_v4"}
  T29 = typedef "Deep_Learning_Toolkit_by_Ngene.lvlib/NNG_WS.ctl" = cluster{"NNG_WS_Mem":T30, "Max_WS_Size":i64}
  T30 = typedef "Deep_Learning_Toolkit_by_Ngene.lvlib/NNg_WS_Mem_DVR.ctl" = refnum<data-value>
  T31 = typedef "Deep_Learning_Toolkit_by_Ngene.lvlib/NN_Layer.ctl" = cluster{"Name":string, "Layer_Data":T32, "Layer_Type":T33, "Dims_In":T25, "Layers_In":T23[], "Dims_Out":T25, "Layers_Out":T23[], "Metrics":T34, "GPU_Data":T35, "mBatch":i32, "NN_Device":T7, "NNg_hdls":T27, "Train?":bool, "Dimty":T36, "RecptField":T37, "Idx":i32}
  T32 = typedef "Deep_Learning_Toolkit_by_Ngene.lvlib/NN_Layer_Data_Refnum.ctl" = refnum<file>
  T33 = typedef "Deep_Learning_Toolkit_by_Ngene.lvlib/NN_Layer_Type.ctl" = enum16{"Input1D", "Input3D", "Conv1D", "Conv2D", "Conv2D_Adv", "MaxPool", "AvgPool", "UpSample", "DropOut3D", "ShortCut", "Concat", "SoftMax3D", "FC", "DropOut", "Softmax", "Flatten", "YOLO_v2", "YOLO_v4", "Activation", "BatchNormalization", "LayerNormalization", "Scale", "Unsupported"}
  T34 = typedef "Deep_Learning_Toolkit_by_Ngene.lvlib/NN_Layer_Metrics.ctl" = cluster{"Data":dbl, "Params":dbl, "Ops":dbl}
  T35 = typedef "Deep_Learning_Toolkit_by_Ngene.lvlib/NNg_Layer_Data_Refnum.ctl" = refnum<file>
  T36 = typedef "Deep_Learning_Toolkit_by_Ngene.lvlib/NN_Layer_Dimty.ctl" = enum16{"1D", "3D"}
  T37 = typedef "Deep_Learning_Toolkit_by_Ngene.lvlib/NN_Layer_RF_State.ctl" = cluster{"Dims":T38, "J":T38}
  T38 = typedef "Deep_Learning_Toolkit_by_Ngene.lvlib/NN_Dims(V,H).ctl" = cluster{"V":i32, "H":i32}
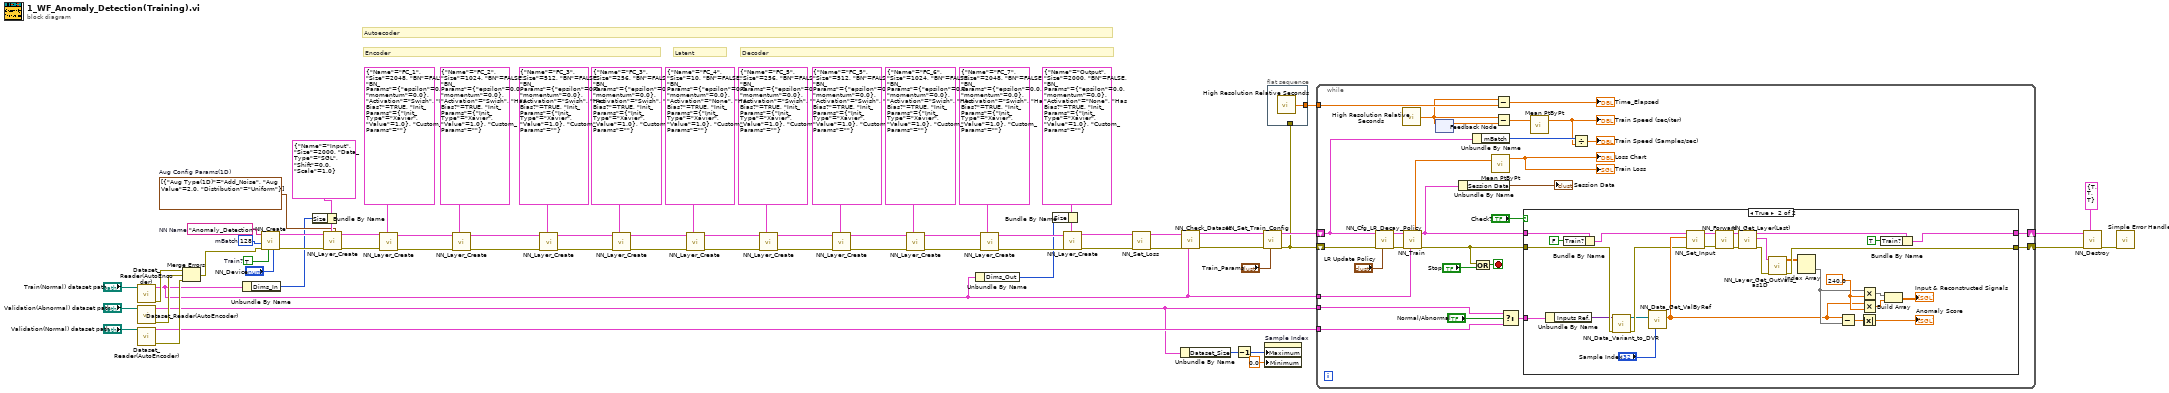
[diagram p0: block diagram]
diagram:
  w18 = T8 [{"Aug Type(1D)"=enum."Add_Noise", "Aug Value"=2.0, "Distribution"=enum."Uniform"}]  # Aug Config Params(1D)
  w60 = TRUE  # Train?
  w64 = 128  # mBatch
  w69 = "Anomaly_Detection"  # NN Name
  # "Latent"
  # "Decoder"
  # "Encoder"
  # "Autoecoder"
  n1 = call "Dataset_Reader(AutoEncoder).vi"("Train dataset path"="Train(Normal) dataset path") -> ("error out"=w7:errorcluster, "Dataset"=w3:T20)  [unwired: 9 in]
  n2 = call "Dataset_Reader(AutoEncoder).vi"("Train dataset path"="Validation(Abnormal) dataset path") -> ("error out"=w8:errorcluster, "Dataset"=w2:T20)  [unwired: 9 in]
  n3 = call "Dataset_Reader(AutoEncoder).vi"("Train dataset path"="Validation(Normal) dataset path") -> ("error out"=w6:errorcluster, "Dataset"=w4:T20)  [unwired: 9 in]
  n4 = Merge Errors(w7, w8, w6) -> (w5:errorcluster)
  n5 = Unbundle By Name(w3) -> ("Dims_In"=w16:i32)
  n6 = call <vilib>:"NN_Create.vi"("NN_Device"="NN_Device", "Train? (false)"=w60, "error in (no error)"=w5, "mBatch (1)"=w64, "Name"=w69) -> ("error out"=w67:errorcluster, "NN out"=w68:T22)  [unwired: 5 in]
  n7 = Bundle By Name(cluster=T17 {"Name"="Input", "Size"=2000, "Data_Type"=enum."SGL", "Shift"=0.0, "Scale"=1.0} ("Input1D_Cfg"), "Size"=w16) -> (w19:T17)
  n8 = call-poly <vilib>:"NN_Layer_Create.vi"("Aug Config Params(1D)"=w18, "Input1D_Cfg"=w19, "error in (no error)"=w67, "NN in"=w68) -> ("error out"=w45:errorcluster, "NN out"=w44:T22)  [unwired: 5 in, 1 out]
  n9 = call-poly <vilib>:"NN_Layer_Create.vi"("FC_Cfg"=T12 {"Name"="FC_1", "Size"=2048, "BN"=FALSE, "BN_Params"={"epsilon"=0.0, "momentum"=0.0}, "Activation"=enum."Swish", "Has Bias?"=TRUE, "Init_Params"={"Init_Type"=enum."Xavier", "Value"=1.0}, "Custom_Params"=""} ("Layer_Config_Params"), "error in (no error)"=w45, "NN in"=w44) -> ("error out"=w40:errorcluster, "NN out"=w41:T22)  [unwired: 6 in, 1 out]
  n10 = call-poly <vilib>:"NN_Layer_Create.vi"("FC_Cfg"=T12 {"Name"="FC_2", "Size"=1024, "BN"=FALSE, "BN_Params"={"epsilon"=0.0, "momentum"=0.0}, "Activation"=enum."Swish", "Has Bias?"=TRUE, "Init_Params"={"Init_Type"=enum."Xavier", "Value"=1.0}, "Custom_Params"=""} ("Layer_Config_Params"), "error in (no error)"=w40, "NN in"=w41) -> ("error out"=w51:errorcluster, "NN out"=w52:T22)  [unwired: 6 in, 1 out]
  n11 = call-poly <vilib>:"NN_Layer_Create.vi"("FC_Cfg"=T12 {"Name"="FC_3", "Size"=512, "BN"=FALSE, "BN_Params"={"epsilon"=0.0, "momentum"=0.0}, "Activation"=enum."Swish", "Has Bias?"=TRUE, "Init_Params"={"Init_Type"=enum."Xavier", "Value"=1.0}, "Custom_Params"=""} ("Layer_Config_Params"), "error in (no error)"=w51, "NN in"=w52) -> ("error out"=w34:errorcluster, "NN out"=w35:T22)  [unwired: 6 in, 1 out]
  n12 = call-poly <vilib>:"NN_Layer_Create.vi"("FC_Cfg"=T12 {"Name"="FC_3", "Size"=256, "BN"=FALSE, "BN_Params"={"epsilon"=0.0, "momentum"=0.0}, "Activation"=enum."Swish", "Has Bias?"=TRUE, "Init_Params"={"Init_Type"=enum."Xavier", "Value"=1.0}, "Custom_Params"=""} ("Layer_Config_Params"), "error in (no error)"=w34, "NN in"=w35) -> ("error out"=w32:errorcluster, "NN out"=w33:T22)  [unwired: 6 in, 1 out]
  n13 = call-poly <vilib>:"NN_Layer_Create.vi"("FC_Cfg"=T12 {"Name"="FC_4", "Size"=10, "BN"=FALSE, "BN_Params"={"epsilon"=0.0, "momentum"=0.0}, "Activation"=enum."None", "Has Bias?"=TRUE, "Init_Params"={"Init_Type"=enum."Xavier", "Value"=1.0}, "Custom_Params"=""} ("Layer_Config_Params"), "error in (no error)"=w32, "NN in"=w33) -> ("error out"=w30:errorcluster, "NN out"=w31:T22)  [unwired: 6 in, 1 out]
  n14 = call-poly <vilib>:"NN_Layer_Create.vi"("FC_Cfg"=T12 {"Name"="FC_5", "Size"=256, "BN"=FALSE, "BN_Params"={"epsilon"=0.0, "momentum"=0.0}, "Activation"=enum."Swish", "Has Bias?"=TRUE, "Init_Params"={"Init_Type"=enum."Xavier", "Value"=1.0}, "Custom_Params"=""} ("Layer_Config_Params"), "error in (no error)"=w30, "NN in"=w31) -> ("error out"=w28:errorcluster, "NN out"=w29:T22)  [unwired: 6 in, 1 out]
  n15 = call-poly <vilib>:"NN_Layer_Create.vi"("FC_Cfg"=T12 {"Name"="FC_5", "Size"=512, "BN"=FALSE, "BN_Params"={"epsilon"=0.0, "momentum"=0.0}, "Activation"=enum."Swish", "Has Bias?"=TRUE, "Init_Params"={"Init_Type"=enum."Xavier", "Value"=1.0}, "Custom_Params"=""} ("Layer_Config_Params"), "error in (no error)"=w28, "NN in"=w29) -> ("error out"=w38:errorcluster, "NN out"=w39:T22)  [unwired: 6 in, 1 out]
  n16 = call-poly <vilib>:"NN_Layer_Create.vi"("FC_Cfg"=T12 {"Name"="FC_6", "Size"=1024, "BN"=FALSE, "BN_Params"={"epsilon"=0.0, "momentum"=0.0}, "Activation"=enum."Swish", "Has Bias?"=TRUE, "Init_Params"={"Init_Type"=enum."Xavier", "Value"=1.0}, "Custom_Params"=""} ("Layer_Config_Params"), "error in (no error)"=w38, "NN in"=w39) -> ("error out"=w46:errorcluster, "NN out"=w47:T22)  [unwired: 6 in, 1 out]
  n17 = Unbundle By Name(w3) -> ("Dims_Out"=w15:i32)
  n18 = call-poly <vilib>:"NN_Layer_Create.vi"("FC_Cfg"=T12 {"Name"="FC_7", "Size"=2048, "BN"=FALSE, "BN_Params"={"epsilon"=0.0, "momentum"=0.0}, "Activation"=enum."Swish", "Has Bias?"=TRUE, "Init_Params"={"Init_Type"=enum."Xavier", "Value"=1.0}, "Custom_Params"=""} ("Layer_Config_Params"), "error in (no error)"=w46, "NN in"=w47) -> ("error out"=w42:errorcluster, "NN out"=w43:T22)  [unwired: 6 in, 1 out]
  n19 = Bundle By Name(cluster=T12 {"Name"="Output", "Size"=2000, "BN"=FALSE, "BN_Params"={"epsilon"=0.0, "momentum"=0.0}, "Activation"=enum."None", "Has Bias?"=TRUE, "Init_Params"={"Init_Type"=enum."Xavier", "Value"=1.0}, "Custom_Params"=""} ("Layer_Config_Params"), "Size"=w15) -> (w17:T12)
  n20 = call-poly <vilib>:"NN_Layer_Create.vi"("FC_Cfg"=w17, "error in (no error)"=w42, "NN in"=w43) -> ("error out"=w25:errorcluster, "NN out"=w63:T22)  [unwired: 6 in, 1 out]
  n21 = call-poly <vilib>:"NN_Set_Loss.vi"("error in (no error)"=w25, "NN in"=w63) -> ("error out"=w24:errorcluster, "NN out"=w26:T22)  [unwired: 8 in]
  n22 = Unbundle By Name(w2) -> ("Dataset_Size"=w14:i32)
  n23 = call-poly <vilib>:"NN_Check_Dataset.vi"("Dataset"=w3, "error in (no error)"=w24, "NN in"=w26) -> ("error out"=w56:errorcluster, "NN out"=w57:T22)  [unwired: 7 in]
  n24 = Decrement(x=w14) -> (x-1=w23:i32)
  n25 = call <vilib>:"NN_Set_Train_Config.vi"("NN_Train_Params"="Train_Params", "error in (no error)"=w56, "NN in"=w57) -> ("error out"=w61:errorcluster, "NN out"=w62:T22)  [unwired: 7 in]
  n26 = property on="Sample Index" class="DigNum (strict)"("Maximum"=w23, "Minimum"=0.0 ("Data Entry Limits:Minimum")) -> ()  [unwired: 2 in, 2 out]
  n27 = flat-sequence {
    tunnel: [w70] -> w66
    tunnel: w61 -> [_]
    frame #0 {
      n28 = call <vilib>:"High Resolution Relative Seconds.vi"() -> ("relative seconds"=w70:dbl)
    }
  }
  n29 = while {
    shift-right: [w84] -> w12
    shift-left: w61 -> [w87]
    shift-right: [w83] -> w13
    shift-left: w62 -> [w88]
    tunnel: w66 -> [w93]
    tunnel: w3 -> [w82]
    tunnel: w4 -> [w74]
    tunnel: w2 -> [w73]
    stop <- w96 stop-if-true
    n30 = call <vilib>:"NN_Cfg_LR_Decay_Policy.vi"("LR_Decay_Params"="LR Update Policy", "error in (no error)"=w87, "NN in"=w88) -> ("error out"=w94:errorcluster, "NN out"=w97:T22)  [unwired: 7 in]
    n31 = call <vilib>:"High Resolution Relative Seconds.vi"() -> ("relative seconds"=w92:dbl)
    n32 = call <vilib>:"NN_Train.vi"("Train Dataset"=w82, "error in (no error)"=w94, "NN in"=w97) -> ("error out"=w85:errorcluster, "NN out"=w86:T22, "Loss"=w95:sgl)  [unwired: 3 in, 3 out]
    n33 = feedback #1() -> (w98:dbl)  [unwired: 1 in]
    n34 = feedback-in #1(w92) -> ()
    n35 = Unbundle By Name(w86) -> ("Session Data"=→"Session Data":T1)
    n36 = Unbundle By Name(w88) -> ("mBatch"=w90:i32)
    n37 = Compound Arithmetic op=OR(w85, "Stop") -> (w96:bool)
    n38 = call <vilib>:"Mean PtByPt.vi"("x"=w95) -> ("mean"=→"Train Loss" →"Loss Chart":dbl)  [unwired: 3 in, 1 out]
    n39 = Subtract(x=w92, y=w93) -> (x-y=→"Time_Elapsed":dbl)
    n40 = Subtract(x=w92, y=w98) -> (x-y=w80:dbl)
    n41 = Select(t=w73, s="Normal/Abnormal", f=w74) -> (s? t:f=w72:T20)
    n42 = case shown="True" "Check?" {
      tunnel: w86 -> [w100 w120]
      tunnel: w85 -> [w99 w128]
      tunnel: [w99 w127] -> w84
      tunnel: [w100 w106] -> w83
      tunnel: w72 -> [_ w113]
      frame False {
      }
      frame True {
        w114 = sgl 240.0 ("x")
        n43 = Unbundle By Name(w113) -> ("Inputs Ref."=w103:variant)
        n44 = Bundle By Name(cluster=w120, "Train?"=FALSE) -> (w121:T22)
        n45 = call-poly <vilib>:"NN_Data_Variant_to_DVR.vi"("error in (no error)"=w128, "Inputs Ref."=w103) -> ("error out"=w102:errorcluster, "DVR(2D_SGL)"=w101:T21)  [unwired: 8 in]
        n46 = call-poly <vilib>:"NN_Data_Get_ValByRef.vi"("index (row)"="Sample Index", "DVR(2D_SGL)"=w101) -> ("Value(1D_SGL)"=w104:sgl[])  [unwired: 6 in, 1 out]
        n47 = call-poly <vilib>:"NN_Set_Input.vi"("error in (no error)"=w102, "Data_In(1D_SGL)"=w104, "NN In"=w121) -> ("error out"=w123:errorcluster, "NN Out"=w122:T22)  [unwired: 7 in]
        n48 = call <vilib>:"NN_Forward.vi"("error in (no error)"=w123, "NN in"=w122) -> ("error out"=w125:errorcluster, "NN out"=w126:T22)  [unwired: 6 in, 2 out]
        n49 = call <vilib>:"NN_Get_Layer(Last).vi"("error in (no error)"=w125, "NN in"=w126) -> ("error out"=w118:errorcluster, "Last_Layer"=w119:T31, "NN out"=w116:T22)  [unwired: 6 in, 1 out]
        n50 = call <vilib>:"NN_Layer_Get_OutVals_as1D.vi"("error in (no error)"=w118, "Layer"=w119) -> ("error out"=w127:errorcluster, "Out(as1D)"=w117:sgl[][])  [unwired: 8 in]
        n51 = Index Array(array=w117) -> (element=w105:sgl[])  [unwired: 2 in]
        n52 = Subtract(x=w104, y=w105) -> (x-y=w111:sgl[])
        n53 = Absolute Value(x=w111) -> (abs(x)=→"Anomaly Score":sgl[])
        n54 = Multiply(x=w105, y=w114) -> (x*y=w112:sgl[])
        n55 = Multiply(x=w104, y=w114) -> (x*y=w110:sgl[])
        n56 = Bundle By Name(cluster=w116, "Train?"=TRUE) -> (w106:T22)
        n57 = Build Array(w112, w110) -> (→"Input & Reconstructed Signals":sgl[][])
      }
    }
    n58 = call <vilib>:"Mean PtByPt.vi"("x"=w80) -> ("mean"=w71:dbl)  [unwired: 3 in, 1 out]
    "Train Speed (sec/iter)" <- w71
    n59 = Divide(x=w90, y=w71) -> (x/y=→"Train Speed (Samples/sec)":dbl)
  }
  n60 = call <vilib>:"NN_Destroy.vi"("Save (T, T, T)"=T19 {"CFG?"=TRUE, "Weights?"=TRUE, "Render?"=TRUE} ("Save_Config"), "error in (no error)"=w12, "NN in"=w13) -> ("error out"=w1:errorcluster)  [unwired: 7 in, 1 out]
  n61 = call <vilib>:"Simple Error Handler.vi"("error in (no error)"=w1) -> ()  [unwired: 4 in, 5 out]
